vi "_VI Helpeks.vi"() -> ()   [LabVIEW 2014]
doc: "::: VI Helpeks :::\nCopyright (c) 2000-2026 Konstantin Shifershteyn. All rights reserved."
uses:
  _VIH Project Manager.llb/VIH Project Tree Typedef - Tree Item Type.ctl
  <vilib>/Utility/miscctls.llb/LVPointTypeDef.ctl
  _VIH Support Library.llb/VIH Utility - APP - Is Value Changed (BOOL).vi
  _VIH Support Library.llb/VIH Utility - APP - Is Value Changed (STR).vi
  <vilib>/Platform/browser.llb/Open URL in Default Browser (path).vi
  <vilib>/Utility/config.llb/Read Key (Path).vi
  <vilib>/Utility/config.llb/Read Key (String).vi
  <resource>/objmgr/DOMUserDefRef.rc
  <vilib>/Utility/config.llb/NI_LVConfig.lvlib
panel:
  in  "%Toolbar_VI_Doc":bool caption="VI Documentation"
  in  "%Toolbar_BuildCHMOpen":bool caption="Open Output CHM File"
  in  "%Toolbar_VI_Edit":bool caption="Edit Source File"
  in  "%Toolbar_BuildCHM":bool caption="Compiled HTML Help"
  in  "%Toolbar_BuildExplore":bool caption="Explore Build Root Folder"
  in  "%Toolbar_Paste":bool caption="Paste File Spec"
  in  "%Toolbar_Copy":bool caption="Copy File Spec"
  in  "%Toolbar_Delete":bool caption="Delete Item"
  in  "%Toolbar_AddGroup":bool caption="Add Group"
  in  "%Toolbar_AddFile":bool caption="Add File"
  in  "%Toolbar_Warning":bool caption="Warning"
  in  "%Toolbar_VI_Term":bool caption="VI Terminal Controls"
  in  "%Toolbar_VI_Open":bool caption="Open Source File"
  in  "%Toolbar_DialogRules":bool caption="Overview File Rules"
  in  "%Toolbar_DialogFiles":bool caption="Overview Project Files"
  in  "%Toolbar_BuildOpen":bool caption="Open Output Help File"
  in  "%Toolbar_BuildLog":bool caption="Open Build Log"
  in  "%Toolbar_BuildSel":bool caption="Build Selected"
  in  "%Toolbar_BuildAll":bool caption="Build All"
  in  "%Toolbar_Save":bool caption="Save Project"
  in  "%Toolbar_Open":bool caption="Open Project"
  in  "%Toolbar_New":bool caption="New Project"
  in  "%%% Show XML":bool
  in  "Tree":string[](tree) caption="Project Tree"
  out "Item Title":string caption="Item Info"
  out "Item Icon":picture
  out "Item Icon BG":string caption="Item Info"
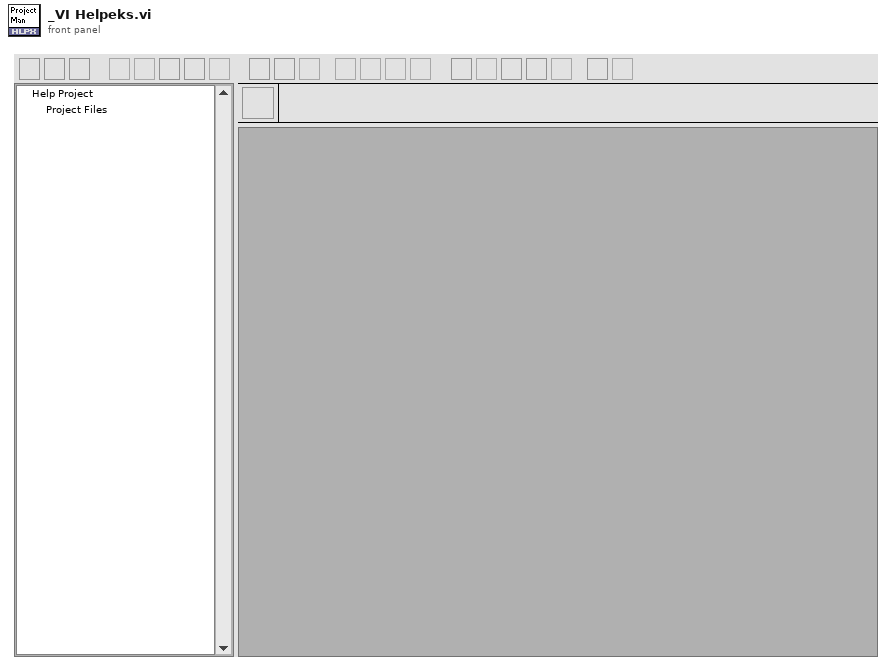
[diagram p1: front panel]
types:
  T1 = typedef "LVPointTypeDef.ctl" = cluster{"Horizontal":i16, "Vertical":i16}
  T2 = typedef "VIH Project Tree Typedef - Tree Item Type.ctl" = enum32{"<Invalid>", "Project", "Proj Files", "Proj Rules", "File Group", "Rule Group", "Any File", "LV Func", ".mnu", ".mnu (dyn)", ".vi", ".vi (dyn)", ".vit", ".vit (dyn)", ".ctl", ".ctl (dyn)", ".ctt", ".ctt (dyn)", "polyVI", "polyVI (dyn)", "expVI", "expVI (dyn)", "HTML", "PolyVI Inst"}
  T3 = cluster{"Product Name":string, "Short Name":string, "Product Version":string, "Release Timestamp":string, "Developer":string, "Copyright":string}
  T4 = enum16{"nop", "Init", "get index", "get symbols"}
  T5 = enum16{"Open", "Close", "Update", "Set Category"}
  T6 = enum32{"edit", "explore", "find", "open", "print"}
  T7 = enum32{"Bad", "Idle", "Run top level", "Running"}
  T8 = enum32{"Invalid", "Default", "Floating", "Floating/Auto-Hide", "Modal"}
  T9 = cluster{"Left Button Key Shortcut":cluster{"Control":bool, "Shift":bool, "Key":string}, "Center Button Key Shortcut":cluster{"Control":bool, "Shift":bool, "Key":string}, "Right Button Key Shortcut":cluster{"Control":bool, "Shift":bool, "Key":string}}
  T10 = enum16{"get", "get all", "set", "Init", "delete", "rename"}
  T11 = enum16{"get", "get all", "set", "Init", "delete"}
  T12 = enum8{"Enabled", "Disabled", "Disabled and Grayed Out"}
  T13 = typedef "eventvkey.ctl" = enum16{"ASCII", "Enter", "Return", "Shift", "Ctrl", "Alt", "Cmd", "Opt", "Caps", "NumLock", "Clear", "Break", "Up", "Down", "Left", "Right", "Insert", "Delete", "Home", "End", "PageUp", "PageDown", "Escape", "Help", "Pause", "ScrollLock", "F1", "F2", "F3", "F4", "F5", "F6", "F7", "F8", "F9", "F10", "F11", "F12", "F13", "F14", "F15", "F16", "F17", "F18", "F19", "F20", "F21", "F22", "F23", "F24", "Play", "VolumeUp", "VolumeDown", "Mute", "Two Byte Char"}
  T14 = cluster{"Shift":bool, "Ctrl":bool, "Alt":bool, "Cmd":bool, "Opt":bool}
  T15 = typedef "VIH HelpGen Typedef - Cluster - Group Rule.ctl" = cluster{"Source Root Dir":path, "Build Root Dir":path, "BuildHelp":T16, "Source Paths":T17, "Target Paths":T18, "VIDscrMode":T19, "MenuDscrMode":T19, "MenuItemIcons":T16, "Control Rules":T20[], "Flags":T22, "Ctl_DscrMode":T19, "Ctl_ClustMembers":T16, "Ctl_EnumValues":T16, "%Comments":string, "PVIIDscrMode":T19, "VIDetailsMode":T19, "ProductInfoMode":T16, "ProductInfoText":string}
  T16 = typedef "VIH HelpGen Typedef - Enum - Default,Enable,Disable.ctl" = enum16{"Default", "Enable", "Disable"}
  T17 = typedef "VIH HelpGen Typedef - Cluster - Group Rule - Source Paths.ctl" = cluster{"CSS Files":path[], "JS Files":path[], "VI Template":path, "Menu Template":path, "PolyVI Template":path}
  T18 = typedef "VIH HelpGen Typedef - Cluster - Group Rule - Target Paths.ctl" = cluster{"HTML Dir":path, "Image Dir":path, "CSS Dir":path, "JS Dir":path}
  T19 = typedef "VIH HelpGen Typedef - Enum - Description Mode.ctl" = enum16{"Default", "Description", "Description1", "Description2", "Custom", "None"}
  T20 = typedef "VIH HelpGen Typedef - Cluster - Control Rule.ctl" = cluster{"CtrlID":string, "CustomRule":bool, "DscrMode":T19, "Description":string, "ClusterMembers":T16, "EnumValues":T16, "EnumValDscr":T21[], "CustomName":string}
  T21 = typedef "VIH HelpGen Typedef - Cluster - Enum Value Info.ctl" = cluster{"Value":ext, "String":string, "Description":string}
  T22 = typedef "VIH HelpGen Typedef - Cluster - Group Rule - Flags.ctl" = cluster{"Override CSS Files":bool, "Override JS Files":bool, "Override Ctl Rules":bool}
  T23 = typedef "LVPoint32TypeDef.ctl" = cluster{"Horizontal":i32, "Vertical":i32}
  T24 = typedef "VIH Project Tree Typedef - Tree Refnum.ctl" = refnum<vi>
  T25 = typedef "lveventtype.ctl" = enum32{"Null", "Timeout", "Annotation Menu Selection", "Annotation Menu Selection?", "App Instance Close", "App Instance Close?", "Autoscale Range Change", "Bookmark Info Change", "Cell Edit", "Cell Edit?", "Cursor Grab", "Cursor Grab?", "Cursor Menu Selection", "Cursor Menu Selection?", "Cursor Move", "Cursor Release", "Data Change", "Direction Change", "Display State Change", "Drag Ended", "Drag Enter", "Drag Leave", "Drag Over", "Drag Source Update", "Drag Starting", "Drag Starting?", "Drop", "Exec State Change", "Key Down", "Key Down?", "Key Repeat", "Key Repeat?", "Key Up", "Listbox Double Click", "Menu Activation?", "Menu Selection (App)", "Menu Selection? (App)", "Menu Selection (User)", "Mouse Down", "Mouse Down?", "Mouse Enter", "Mouse Leave", "Mouse Move", "Mouse Up", "Mouse Wheel", "NI Security User Change (App)", "Pane Size", "Panel Close", "Panel Close?", "Panel Resize", "Plot Attribute Change", "Scale Range Change", "Shortcut Menu Activation?", "Shortcut Menu Selection (App)", "Shortcut Menu Selection? (App)", "Shortcut Menu Selection (User)", "Tree Double Click", "Tree Drag", "Tree Drag?", "Tree Drop", "Tree Drop?", "Tree Item Close", "Tree Item Close?", "Tree Item Open", "Tree Item Open?", "User Event", "Value Change"}
  T26 = cluster{"Show Window":bool, "Show Progress":bool, "Generate HTML":bool, "Generate HHP":bool, "Generate CHM":bool}
  T27 = cluster{"ShowQuickTips":bool, "NextQuickTip":i32, "FastLoadVI":bool, "EditPrgs ":cluster{"FileExtension":string, "CustProgram":path, "UseCustPrg":bool}[]}
  T28 = typedef "NI_LVConfig.lvlib/Config Data RefNum.ctl" = refnum<k1>
  T29 = cluster{"FileExtension":string, "CustProgram":path, "UseCustPrg":bool}[]
  T30 = typedef "VIH HelpGen Typedef - Cluster - File Rule.ctl" = cluster{"OutName":string, "BuildHelp":T16, "Source Paths":T31, "Target Paths":T32, "DscrMode":T19, "Description":string, "Control Rules":T20[], "Flags":T22, "Ctl_DscrMode":T19, "Ctl_ClustMembers":T16, "Ctl_EnumValues":T16, "MenuItemIcons":T16, "%Comments":string, "DetailsMode":T19, "DetailsText":string, "ProductInfoMode":T16, "ProductInfoText":string}
  T31 = typedef "VIH HelpGen Typedef - Cluster - File Rule - Source Paths.ctl" = cluster{"CSS Files":path[], "JS Files":path[], "Html Template":path}
  T32 = typedef "VIH HelpGen Typedef - Cluster - File Rule - Target Paths.ctl" = cluster{"HTML Dir":path, "Image Dir":path, "CSS Dir":path, "JS Dir":path}
  T33 = typedef "VIH HelpGen Typedef - Palette - Item Type Enum.ctl" = enum32{"<Invalid>", "<unknown>", "VI", "Menu", "LV Func", "Express VI", "Poly VI", "CTL", "HTML"}
  T34 = typedef "VIH - CHM Project - HHP Generation Params Cluster.ctl" = cluster{"HHP_Template":enum16{"default", "custom"}, "HHP_Template_CustomPath":path, "HHP_Target":enum16{"default", "custom"}, "HHP_Target_CustomPath":path, "HHP_CreateTOC":bool, "HHP_CreateIDX":bool, "HHP_DefaultTopic":enum16{"auto", "custom"}, "HHP_DefaultTopic_CustomPath":path, "CHM_Filename":path, "HHP_AutoBuild":bool, "CHM_AutoBuild":bool}
  T35 = enum16{"Left Button", "Center Button", "Right Button", "Window Close"}
  T36 = cluster{"DOM doc":refnum<k20>, "Project":refnum<k20>, "Files":refnum<k20>}
  T37 = typedef "VIH HelpGen Typedef - Product Info Cluster.ctl" = cluster{"ProductName":string, "Version":string, "Author":string, "Company":string, "Copyright":string, "Website":string, "Email":string, "AddInfo":string}
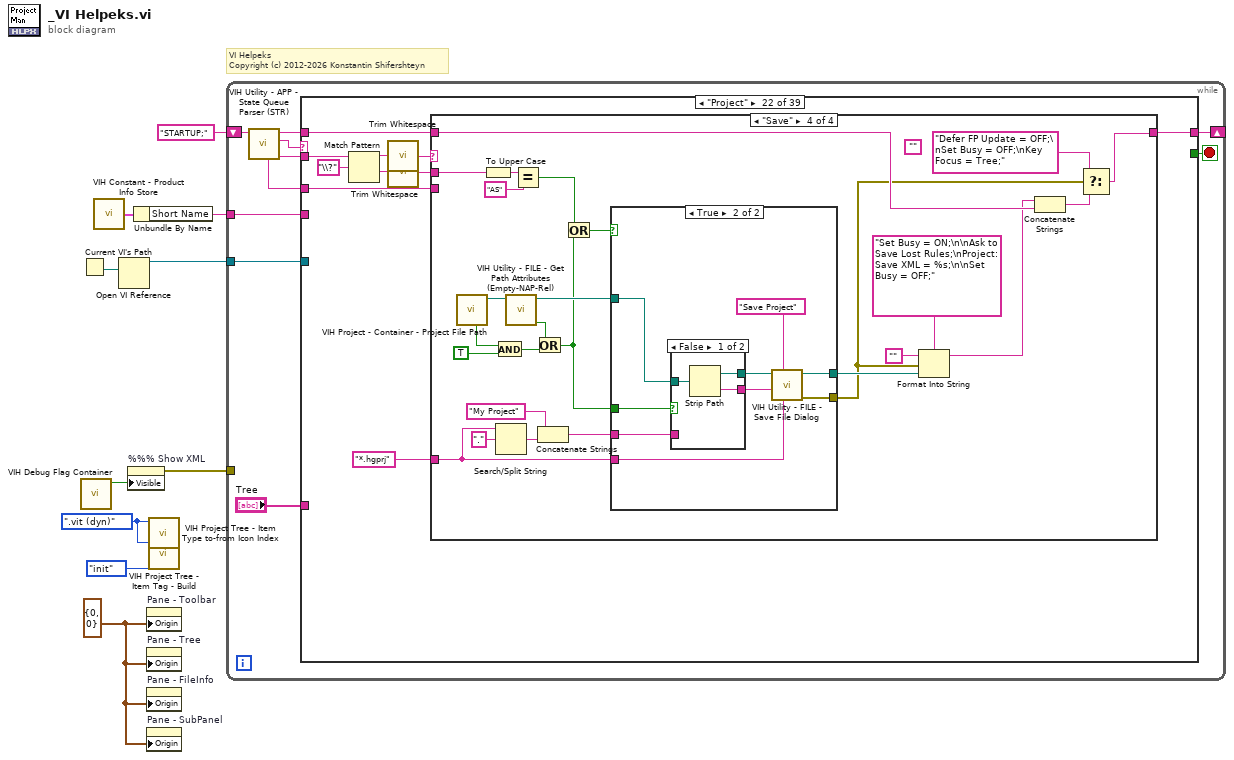
[diagram p0: block diagram]
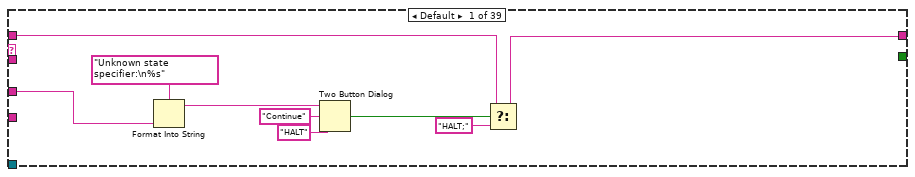
[diagram p2: hidden frame]
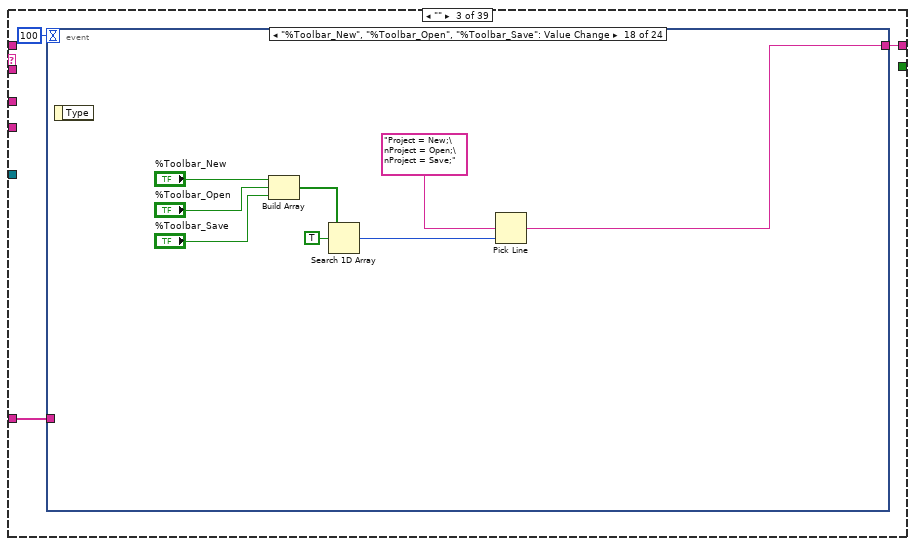
[diagram p4: hidden frame]
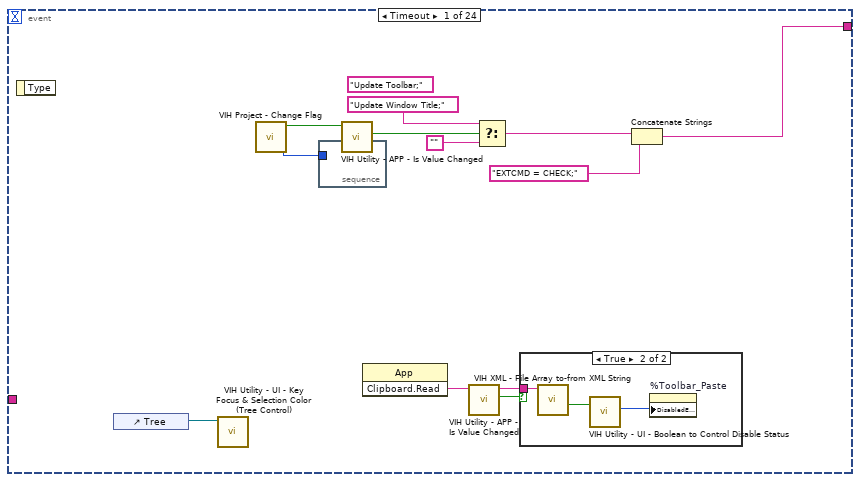
[diagram p5: hidden frame]
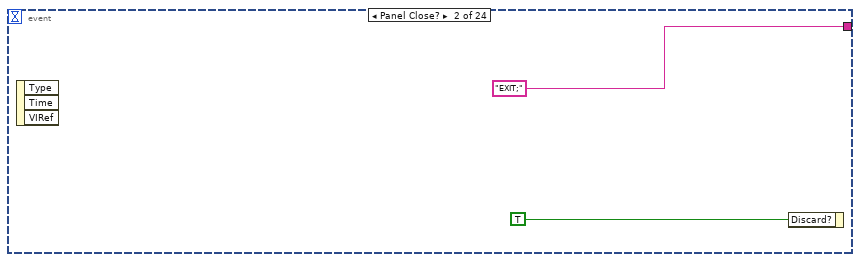
[diagram p7: hidden frame]
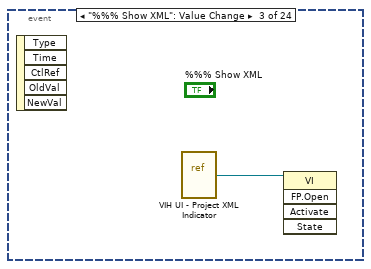
[diagram p8: hidden frame]
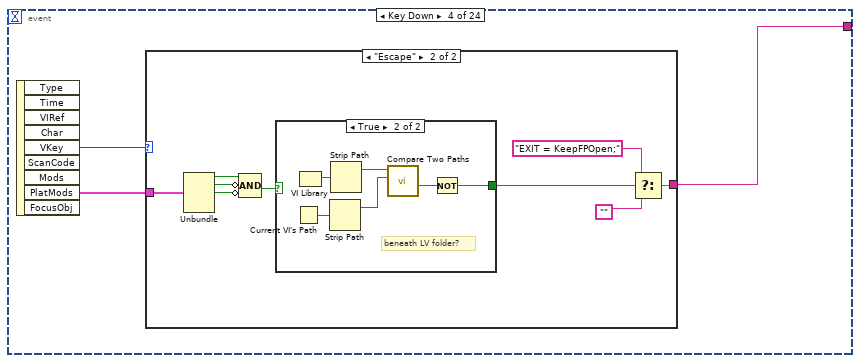
[diagram p9: hidden frame]
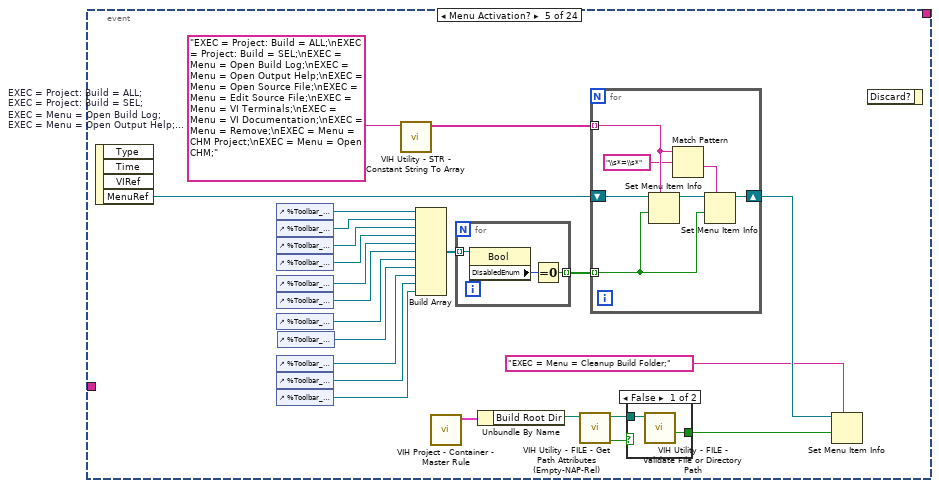
[diagram p12: hidden frame]
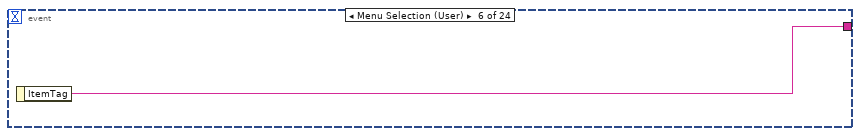
[diagram p14: hidden frame]
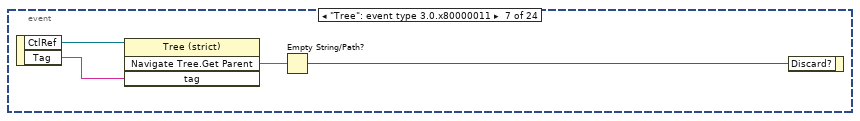
[diagram p15: hidden frame]
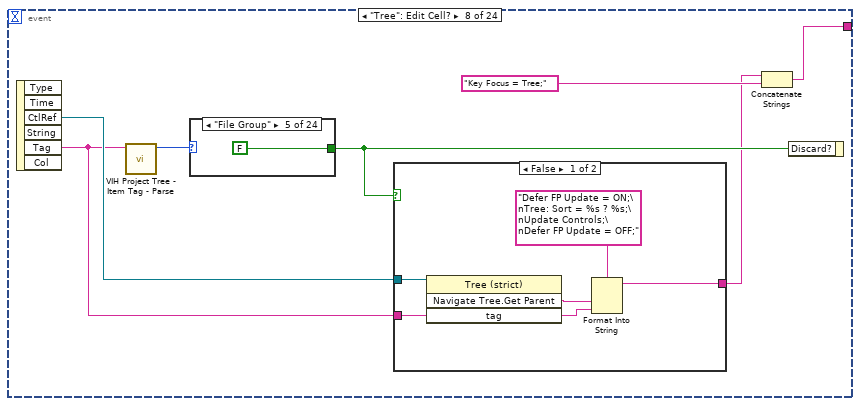
[diagram p16: hidden frame]
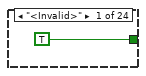
[diagram p18: hidden frame]
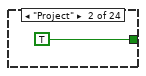
[diagram p19: hidden frame]
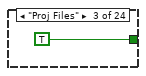
[diagram p20: hidden frame]
diagram:
  w5 = T1 {"Horizontal"=0, "Vertical"=0} ("Origin")
  w8 = VIH_Project_Tree_Typedef_-_Tree_Item_Type.".vit (dyn)" ("Item Type")
  # "VI Helpeks\nCopyright (c) 2012-2026 Konstantin Shifershteyn"
  n1 = Current VI's Path() -> (path=w2:path)
  n2 = call "VIH Debug Flag Container.vi"() -> ("Debug Mode"=w4:bool)  [unwired: 11 in]
  n3 = call "VIH Constant - Product Info Store.vi"() -> ("Product Info"=w6:T3)
  n4 = Open VI Reference(vi path=w2) -> (vi reference=w1:refnum<vi>)  [unwired: 5 in, 1 out]
  n5 = property on="%%% Show XML" class="Bool"("Visible"=w4) -> (error out=w3:errorcluster)  [unwired: 2 in, 1 out]
  n6 = Unbundle By Name(w6) -> ("Short Name"=w7:string)
  n7 = property on="Pane - Toolbar" class="Pane"("Origin"=w5) -> ()  [unwired: 2 in, 2 out]
  n8 = property on="Pane - Tree" class="Pane"("Origin"=w5) -> ()  [unwired: 2 in, 2 out]
  n9 = property on="Pane - FileInfo" class="Pane"("Origin"=w5) -> ()  [unwired: 2 in, 2 out]
  n10 = property on="Pane - SubPanel" class="Pane"("Origin"=w5) -> ()  [unwired: 2 in, 2 out]
  n11 = call "VIH Project Tree - Item Type to-from Icon Index.vi"("Item Type"=w8) -> ()  [unwired: 10 in, 1 out]
  n12 = call "VIH Project Tree - Item Tag - Build.vi"("cmd (build)"=enum16{"build", "init"}."init", "Item Type"=w8) -> ()  [unwired: 8 in, 2 out]
  n13 = while {
    shift-right: [w17] -> _
    shift-left: "STARTUP;" -> [w20]
    tunnel: w7 -> [w12]
    tunnel: w3 -> [_]
    tunnel: w1 -> [w11]
    stop <- w15 stop-if-true
    n14 = call "VIH Utility - APP - State Queue Parser (STR).vi"("input queue"=w20) -> ("state parameters"=w14:string, "state"=w19:string, "remained queue"=w16:string, "complete state specifier"=w18:string)  [unwired: 5 in]
    n15 = case shown="\"Project\"" w19 {
      tunnel: w18 -> [w28 _ _ _ _ _ _ w438 _ _ _ _ _ _ _ w624 _ _ _ _ _ w1140 _ _ _ _ _ _ _ _ _ _ _ _ _ _ _ _ _]
      tunnel: [w22 w30 w33 w364 w397 w406 w418 w437 w545 w574 w583 w598 w608 w614 w616 w623 w1082 w1086 w1091 w1109 w1135 w1137 w1209 w1215 w1285 w1329 w1340 w1351 w1473 w1491 w1502 w1551 w1570 w1580 w1595 w1605 w1615 w1666 w1719] -> w17
      tunnel: w16 -> [w23 w30 _ w365 w398 w406 w418 w436 _ w574 w583 w598 w608 w614 w616 w630 w1081 w1086 w1092 w1116 w1135 w1136 w1210 w1216 w1286 w1330 w1340 w1369 w1476 w1491 w1502 w1551 w1570 w1582 w1595 w1605 w1621 w1666 w1732]
      tunnel: [_ _ _ _ _ _ _ _ _ TRUE _ _ _ _ _ _ _ _ _ _ _ _ _ _ _ _ _ _ _ _ _ _ _ _ _ _ _ _ _] -> w15
      tunnel: w14 -> [_ _ _ _ _ w402 w416 w441 w544 w572 _ w597 w607 w612 w615 w629 w1084 _ _ _ _ w1145 w1205 w1212 w1283 w1327 w1337 w1367 _ _ _ _ w1567 _ _ _ w1616 _ w1725]
      tunnel: "Tree" -> [_ _ w31 _ _ _ _ _ _ _ _ _ _ _ _ w619 _ _ _ _ _ _ _ _ _ _ _ w1368 _ _ _ _ _ _ _ _ _ w1655 _]
      tunnel: w12 -> [_ _ _ _ _ _ _ _ _ w570 _ _ _ _ _ _ _ _ _ _ _ _ _ _ w1253 _ _ w1344 _ _ _ _ _ _ _ w1601 _ _ _]
      tunnel: w11 -> [_ _ _ _ _ w407 _ _ _ w560 _ _ _ _ _ _ _ _ _ _ _ _ _ _ _ _ _ _ _ _ _ _ _ _ _ _ _ _ _]
      frame Default {
        n16 = Format Into String(format string="Unknown state specifier:\n%s", w28) -> (resulting string=w27:string)  [unwired: 2 in, 1 out]
        n17 = Two Button Dialog(message=w27, 1:"HALT" ("F button name (\"Cancel\")"), 2:"Continue" ("T button name (\"OK\")")) -> (T button?=w24:bool)
        n18 = Select(t=w23, s=w24, f="HALT;") -> (s? t:f=w22:string)
      }
      frame "#" {
      }
      frame "" {
        n19 = event shown="[17] \"%Toolbar_New\", \"%Toolbar_Open\", \"%Toolbar_Save\": Value Change" {
          selector: _ -> [_ _ _ _ _ _ _ _ _ _ _ _ _ _ _ _ _ _ _ _ _ _ _ _]
          dyn-events: _ -> [_ _ _ _ _ _ _ _ _ _ _ _ _ _ _ _ _ _ _ _ _ _ _ _]
          timeout: 100 -> [_ _ _ _ _ _ _ _ _ _ _ _ _ _ _ _ _ _ _ _ _ _ _ _]
          tunnel: [w35 "EXIT;" _ w52 _ w105 _ w110 _ _ w195 "Defer FP Update = ON;\nUpdate Controls;\nDefer FP Update = OFF;" ("format string") "Update Controls;\nKey Focus = Tree;" w260 "Key Focus = Tree;" ("format string") w279 w281 w307 w316 w327 w336 w343 w353 "Menu = WARNING;"] -> w33
          tunnel: w31 -> [_ _ _ _ _ _ _ _ _ _ _ _ _ _ _ _ _ _ _ _ _ _ _ _]
          event Timeout {
            (unwired) "Update Toolbar;"
            n20 = event-data() -> ()  [unwired: 1 in, 1 out]
            n21 = control-ref of="Tree"() -> (w45:refnum<vi>)
            n22 = call "VIH Utility - UI - Key Focus & Selection Color (Tree Control).vi"("Tree Refnum"=w45) -> ()  [unwired: 8 in, 3 out]
            n23 = call "VIH Project - Change Flag.vi"() -> ("Counter"=w39:i32, "Flag"=w40:bool)  [unwired: 10 in]
            n24 = stacked-sequence {
              tunnel: w39 -> [_]
              frame #0 {
              }
            }
            n25 = call-poly "VIH Utility - APP - Is Value Changed.vi"("Value"=w40) -> ("Changed"=w44:bool)  [unwired: 5 in, 1 out]
            n26 = invoke class="App" method="Clipboard.Read"() -> ("Read Clipbrd"=w36:string)  [unwired: 3 in, 2 out]
            n27 = call-poly "VIH Utility - APP - Is Value Changed.vi"("Value"=w36) -> ("Changed"=w38:bool, "dup Value"=w37:string)  [unwired: 5 in]
            n28 = Select(t="Update Window Title;", s=w44, f="") -> (s? t:f=w41:string)
            n29 = case shown="True" w38 {
              tunnel: w37 -> [_ w46]
              frame False {
              }
              frame True {
                n30 = call "VIH XML - File Array to-from XML String.vi"("XML in"=w46) -> ("available"=w47:bool)  [unwired: 7 in, 3 out]
                n31 = call "VIH Utility - UI - Boolean to Control Disable Status.vi"("Status in"=w47) -> ("Control Disable if False"=w48:u8)  [unwired: 3 in, 1 out]
                n32 = property on="%Toolbar_Paste" class="Bool"("DisabledEnum"=w48) -> ()  [unwired: 2 in, 2 out]
              }
            }
            n33 = Concatenate Strings(w41, "EXTCMD = CHECK;") -> (w35:string)
          }
          event Panel Close? {
            n34 = event-data() -> ()  [unwired: 1 in, 3 out]
            n35 = event-data("Discard?"=TRUE) -> ()  [unwired: 1 in, 1 out]
          }
          event "%%% Show XML": Value Change {
            n36 = event-data() -> ()  [unwired: 1 in, 5 out]
            n37 = vi-ref "VIH UI - Project XML Indicator.vi"() -> (w51:refnum<vi>)
            n38 = invoke class="VI" method="FP.Open"(reference=w51) -> ()  [unwired: 4 in, 5 out]
          }
          event Key Down {
            n39 = event-data() -> ("VKey"=w54:T13, "PlatMods"=w53:T14)  [unwired: 1 in, 7 out]
            n40 = case shown="\"Escape\"" w54 {
              tunnel: w53 -> [_ w63]
              tunnel: [_ w57] -> w52
              frame Default {
              }
              frame "Escape" {
                n41 = Unbundle(w63) -> ("Shift"=w62:bool, "Ctrl"=w61:bool, "Alt"=w60:bool)  [unwired: 2 out]
                n42 = Compound Arithmetic op=AND(w62, invert w61, invert w60) -> (w55:bool)
                n43 = case shown="True" w55 {
                  tunnel: [_ w64] -> w56
                  frame False {
                  }
                  frame True {
                    # "beneath LV folder?"
                    n44 = Current VI's Path() -> (path=w66:path)
                    n45 = VI Library() -> (path=w69:path)
                    n46 = Strip Path(path=w66) -> (stripped path=w67:path)  [unwired: 1 out]
                    n47 = Strip Path(path=w69) -> (stripped path=w68:path)  [unwired: 1 out]
                    n48 = call <vilib>:"Compare Two Paths.vi"("Path 2"=w67, "Path 1"=w68) -> ("Path 2 Relative to Path 1?"=w65:bool)  [unwired: 6 in, 3 out]
                    n49 = Not(x=w65) -> (.not. x?=w64:bool)
                  }
                }
                n50 = Select(t="EXIT = KeepFPOpen;", s=w56, f="") -> (s? t:f=w57:string)
              }
            }
          }
          event Menu Activation? {
            w85 = "EXEC = Project: Build = ALL;\nEXEC = Project: Build = SEL;\nEXEC = Menu = Open Build Log;\nEXEC = Menu = Open Output Help;\nEXEC = Menu = Open Source File;\nEXEC = Menu = Edit Source File;\nEXEC = Menu = VI Terminals;\nEXEC = Menu = VI Documentation;\nEXEC = Menu = Remove;\nEXEC = Menu = CHM Project;\nEXEC = Menu = Open CHM;"  # EXEC = Project: Build = ALL; EXEC = Project: Build = SEL; EXEC = Menu = Open Build Log; EXEC = Menu = Open Output Help; EXEC = Menu = Open Source File; EXEC = Menu = Edit Source File; EXEC = Menu = VI Terminals; EXEC = Menu = VI Documentation; EXEC = Menu = Remove; EXEC = Menu = CHM Project; EXEC = Menu = Open CHM;
            n51 = event-data() -> ("MenuRef"=w92:refnum<k9>)  [unwired: 1 in, 3 out]
            n52 = control-ref of="%Toolbar_BuildAll"() -> (w91:refnum<vi>)
            n53 = control-ref of="%Toolbar_BuildSel"() -> (w90:refnum<vi>)
            n54 = control-ref of="%Toolbar_BuildLog"() -> (w89:refnum<vi>)
            n55 = control-ref of="%Toolbar_BuildOpen"() -> (w88:refnum<vi>)
            n56 = control-ref of="%Toolbar_VI_Open"() -> (w87:refnum<vi>)
            n57 = control-ref of="%Toolbar_VI_Edit"() -> (w72:refnum<vi>)
            n58 = control-ref of="%Toolbar_VI_Term"() -> (w86:refnum<vi>)
            n59 = control-ref of="%Toolbar_Delete"() -> (w82:refnum<vi>)
            n60 = control-ref of="%Toolbar_BuildCHM"() -> (w80:refnum<vi>)
            n61 = control-ref of="%Toolbar_BuildCHMOpen"() -> (w71:refnum<vi>)
            n62 = control-ref of="%Toolbar_VI_Doc"() -> (w70:refnum<vi>)
            n63 = call "VIH Utility - STR - Constant String To Array.vi"("String in"=w85) -> ("Array out"=w84:string[])  [unwired: 10 in]
            n64 = Build Array(w91, w90, w89, w88, w87, w72, w86, w70, w82, w80, w71) -> (w83:refnum<vi>[])
            n65 = call "VIH Project - Container - Master Rule.vi"() -> ("Rule out"=w76:T15)  [unwired: 11 in]
            n66 = for {
              tunnel: w83 -> [w96] mode=indexing
              tunnel: [w95] -> w81 mode=indexing
              n67 = property class="Bool"(reference=w96) -> ("DisabledEnum"=w97:T12)  [unwired: 1 in, 2 out]
              n68 = Equal To 0?(x=w97) -> (x = 0?=w95:bool)
            }
            n69 = Unbundle By Name(w76) -> ("Build Root Dir"=w77:path)
            n70 = call "VIH Utility - FILE - Get Path Attributes (Empty-NAP-Rel).vi"("Path"=w77) -> ("Not A Path or Empty path"=w79:bool, "dup Path"=w78:path)  [unwired: 6 in, 3 out]
            n71 = for {
              tunnel: w84 -> [w102] mode=indexing
              tunnel: w81 -> [w99] mode=indexing
              shift-right: [w98] -> w75
              shift-left: w92 -> [w104]
              n72 = Set Menu Item Info(7:w102, 9:w99, 11:w104) -> (3:w103:refnum<k9>)  [unwired: 4 in, 1 out]
              n73 = Match Pattern(string=w102, regular expression="\\s*=\\s*") -> (after substring=w100:string)  [unwired: 1 in, 3 out]
              n74 = Set Menu Item Info(7:w100, 9:w99, 11:w103) -> (3:w98:refnum<k9>)  [unwired: 4 in, 1 out]
            }
            n75 = case shown="False" w79 {
              tunnel: w78 -> [w94 _]
              tunnel: [w93 _] -> w73
              frame False {
                n76 = call "VIH Utility - FILE - Validate File or Directory Path.vi"("Path"=w94) -> ("directory"=w93:bool)  [unwired: 6 in, 4 out]
              }
              frame True {
              }
            }
            n77 = Set Menu Item Info(7:"EXEC = Menu = Cleanup Build Folder;", 9:w73, 11:w75) -> ()  [unwired: 4 in, 2 out]
            n78 = event-data() -> ()  [unwired: 2 in, 1 out]
          }
          event Menu Selection (User) {
            n79 = event-data() -> ("ItemTag"=w105:string)  [unwired: 1 in]
          }
          event "Tree": event type 3.0.x80000011 {
            n80 = event-data() -> ("CtlRef"=w109:refnum<vi>, "Tag"=w108:string)  [unwired: 1 in]
            n81 = invoke class="Tree (strict)" method="Navigate Tree.Get Parent"(reference=w109, "tag"=w108) -> ("Navigate Tree:Get Parent"=w107:string)  [unwired: 2 in, 3 out]
            n82 = Empty String/Path?(string/path=w107) -> (empty?=w106:bool)
            n83 = event-data("Discard?"=w106) -> ()  [unwired: 1 in, 1 out]
          }
          event "Tree": Edit Cell? {
            n84 = event-data() -> ("CtlRef"=w114:refnum<vi>, "Tag"=w113:string)  [unwired: 1 in, 4 out]
            n85 = call "VIH Project Tree - Item Tag - Parse.vi"("Tree Item Tag"=w113) -> ("Item Type"=w116:T2)  [unwired: 8 in, 2 out]
            n86 = case shown="\"File Group\"" w116 {
              tunnel: [TRUE TRUE TRUE TRUE FALSE FALSE TRUE TRUE TRUE TRUE TRUE TRUE TRUE TRUE TRUE TRUE TRUE TRUE TRUE TRUE TRUE TRUE TRUE TRUE] -> w115
              frame "<Invalid>" {
              }
              frame "Project" {
              }
              frame "Proj Files" {
              }
              frame "Proj Rules" {
              }
              frame "File Group" {
              }
              frame "Rule Group" {
              }
              frame "Any File" {
              }
              frame "LV Func" {
              }
              frame ".mnu" {
              }
              frame ".mnu (dyn)" {
              }
              frame ".vi" {
              }
              frame ".vi (dyn)" {
              }
              frame ".vit" {
              }
              frame ".vit (dyn)" {
              }
              frame ".ctl" {
              }
              frame ".ctl (dyn)" {
              }
              frame ".ctt" {
              }
              frame ".ctt (dyn)" {
              }
              frame "polyVI" {
              }
              frame "polyVI (dyn)" {
              }
              frame "expVI" {
              }
              frame "expVI (dyn)" {
              }
              frame "HTML" {
              }
              frame "PolyVI Inst" {
              }
            }
            n87 = case shown="False" w115 {
              tunnel: w114 -> [w121 _]
              tunnel: w113 -> [w117 _]
              tunnel: [w118 _] -> w111
              frame False {
                n88 = invoke class="Tree (strict)" method="Navigate Tree.Get Parent"(reference=w121, "tag"=w117) -> ("Navigate Tree:Get Parent"=w119:string)  [unwired: 2 in, 3 out]
                n89 = Format Into String(format string="Defer FP Update = ON;\nTree: Sort = %s ? %s;\nUpdate Controls;\nDefer FP Update = OFF;", w119, w117) -> (resulting string=w118:string)  [unwired: 2 in, 1 out]
              }
              frame True {
              }
            }
            n90 = Concatenate Strings(w111, "Key Focus = Tree;") -> (w110:string)
            n91 = event-data("Discard?"=w115) -> ()  [unwired: 1 in, 1 out]
          }
          event "Tree": Drag Starting? {
            n92 = event-data() -> ("CtlRef"=w149:refnum<vi>)  [unwired: 1 in, 8 out]
            n93 = property class="Tree (strict)"(reference=w149) -> ("Value"=w146:string[])  [unwired: 1 in, 2 out]
            n94 = for {
              tunnel: [w154] -> w150 mode=indexing
              tunnel: w146 -> [w153] mode=indexing
              n95 = call "VIH Project Tree - Item Tag - Parse.vi"("Tree Item Tag"=w153) -> ("Item File Path"=w151:path, "Item Type"=w152:T2)  [unwired: 8 in, 1 out]
              n96 = case shown="\"PolyVI Inst\"" w152 {
                tunnel: [w155 FALSE FALSE FALSE TRUE TRUE TRUE FALSE TRUE FALSE TRUE FALSE TRUE FALSE TRUE FALSE TRUE FALSE TRUE FALSE TRUE FALSE TRUE FALSE] -> w154
                tunnel: w151 -> [w157 _ _ _ _ _ _ _ _ _ _ _ _ _ _ _ _ _ _ _ _ _ _ _]
                frame "<Invalid>" {
                  (unwired) FALSE
                  n97 = Empty String/Path?(string/path=w157) -> (empty?=w156:bool)
                  n98 = Not(x=w156) -> (.not. x?=w155:bool)
                }
                frame "Project" {
                }
                frame "Proj Files" {
                }
                frame "Proj Rules" {
                }
                frame "File Group" {
                }
                frame "Rule Group" {
                }
                frame "Any File" {
                }
                frame "LV Func" {
                }
                frame ".mnu" {
                }
                frame ".mnu (dyn)" {
                }
                frame ".vi" {
                }
                frame ".vi (dyn)" {
                }
                frame ".vit" {
                }
                frame ".vit (dyn)" {
                }
                frame ".ctl" {
                }
                frame ".ctl (dyn)" {
                }
                frame ".ctt" {
                }
                frame ".ctt (dyn)" {
                }
                frame "polyVI" {
                }
                frame "polyVI (dyn)" {
                }
                frame "expVI" {
                }
                frame "expVI (dyn)" {
                }
                frame "HTML" {
                }
                frame "PolyVI Inst" {
                }
              }
            }
            n99 = And Array Elements(Boolean array=w150) -> (logical AND=w148:bool)
            n100 = Not(x=w148) -> (.not. x?=w147:bool)
            n101 = event-data("Discard?"=w147) -> ()  [unwired: 1 in, 1 out]
          }
          event "Tree": event type 3.0.xa000003a {
            n102 = event-data() -> ("CtlRef"=w188:refnum<vi>, "Coords"=w189:T23)  [unwired: 1 in, 3 out]
            n103 = invoke class="Tree (strict)" method="Point To Row Column"(reference=w188, "Point"=w189) -> (reference out=w187:refnum<vi>, "InBounds"=w182:bool, "Tag"=w184:string)  [unwired: 6 in, 5 out]
            n104 = property class="Tree (strict)"(reference=w187) -> (reference out=w186:refnum<vi>, "Value"=w185:string[])  [unwired: 1 in, 1 out]
            n105 = call "VIH Project Tree - Is Drop Allowed.vi"("Target Item Tag"=w184, "Source Item Tags"=w185, "Tree Refnum"=w186) -> ("Drop Allowed"=w183:bool)  [unwired: 6 in, 2 out]
            n106 = And(x=w183, y=w182) -> (x .and. y?=w181:bool)
            n107 = event-data("Accepted?"=w181) -> ()  [unwired: 1 in, 1 out]
          }
          event "Tree": Drop {
            n108 = event-data() -> ("CtlRef"=w197:refnum<vi>, "Coords"=w198:T23)  [unwired: 1 in, 3 out]
            n109 = invoke class="Tree (strict)" method="Point To Row Column"(reference=w197, "Point"=w198) -> (reference out=w193:refnum<vi>, "Tag"=w192:string)  [unwired: 6 in, 6 out]
            n110 = property class="Tree (strict)"(reference=w193) -> (reference out=w194:refnum<vi>, "Value"=w190:string[])  [unwired: 1 in, 1 out]
            n111 = call "VIH Project Tree - Is Drop Allowed.vi"("Target Item Tag"=w192, "Source Item Tags"=w190, "Tree Refnum"=w194) -> ("Drop Allowed"=w191:bool)  [unwired: 6 in, 2 out]
            n112 = case shown="True" w191 {
              tunnel: w197 -> [_ w201]
              tunnel: w192 -> [_ w204]
              tunnel: [_ w205] -> w195
              tunnel: w190 -> [_ w203]
              frame False {
              }
              frame True {
                n113 = call "VIH Project Tree - Defer Panel Updates.vi"("Defer Panel Updates (F)"=TRUE, "Project Tree"=w201) -> ("dup Project Tree"=w200:T24)  [unwired: 7 in, 2 out]
                n114 = Index Array(array=w203) -> (element=w202:string)  [unwired: 1 in]
                n115 = for {
                  tunnel: w204 -> [w210]
                  shift-right: [w211] -> w207
                  shift-left: w200 -> [w213]
                  tunnel: w203 -> [w209] mode=indexing
                  n116 = invoke class="Tree (strict)" method="Edit Tree Items.Move Item"(reference=w213, "tag"=w209, "New Parent"=w210, "Carry Children"=TRUE) -> (reference out=w211:T24)  [unwired: 3 in, 6 out]
                }
                n117 = invoke class="Tree (strict)" method="Open/Close.Item"(reference=w207, "tag"=w204, "Open"=TRUE) -> ()  [unwired: 2 in, 5 out]
                n118 = Format Into String(format string="Defer FP Update = ON;\nTree: Sort = %s ? %s;\nUpdate Controls;\nDefer FP Update = OFF;", w204, w202) -> (resulting string=w205:string)  [unwired: 2 in, 1 out]
              }
            }
            n119 = event-data("Accepted?"=FALSE) -> ()  [unwired: 1 in, 1 out]
          }
          event "Tree": Value Change {
            n120 = event-data() -> ("CtlRef"=w217:refnum<vi>, "NewVal"=w216:string[])  [unwired: 1 in, 3 out]
            n121 = Array Size(array=w216) -> (size(s)=w214:i32)
            n122 = case shown="2.." w214 {
              selector: w214 -> [_ w218]
              tunnel: w217 -> [_ w224]
              tunnel: w216 -> [_ w223]
              frame ..1 {
              }
              frame 2.. {
                n123 = Decrement(x=w218) -> (x-1=w222:i32)
                n124 = Index Array(array=w223, index=w222) -> (element=w219:string)
                n125 = property class="Tree (strict)"(reference=w224, "Active Item Tag"=w219) -> (reference out=w220:refnum<vi>, "Indent Level"=w221:i32)  [unwired: 1 in, 1 out]
                n126 = case shown="0, 1" w221 {
                  tunnel: w220 -> [w227 _]
                  tunnel: w219 -> [w226 _]
                  frame 0, 1 {
                    n127 = Build Array(w226) -> (w225:string[])
                    n128 = property class="Tree (strict)"(reference=w227, "Value"=w225) -> ()  [unwired: 1 in, 2 out]
                  }
                  frame Default {
                  }
                }
              }
            }
          }
          event "Tree": Shortcut Menu Activation? {
            (unwired) "Key Focus = Tree;"
            n129 = event-data() -> ("Type"=w230:T25, "CtlRef"=w238:refnum<vi>, "MenuRef"=w237:refnum<k9>, "Coords"=w229:T23)  [unwired: 1 in, 1 out]
            n130 = invoke class="Tree (strict)" method="Point To Row Column"(reference=w238, "Point"=w229) -> (reference out=w231:refnum<vi>, "InBounds"=w235:bool, "Tag"=w234:string)  [unwired: 6 in, 5 out]
            n131 = Select(t=w234, s=w235, f="") -> (s? t:f=w232:string)
            n132 = case shown="Default" w232 {
              selector: w232 -> [w243 _]
              tunnel: w237 -> [w244 _]
              tunnel: [_ TRUE] -> w236
              tunnel: w231 -> [w240 _]
              tunnel: w230 -> [w245 _]
              tunnel: w229 -> [w242 _]
              frame Default {
                n133 = property class="Tree (strict)"(reference=w240) -> (reference out=w246:refnum<vi>, "Value"=w248:string[])  [unwired: 1 in, 1 out]
                n134 = Search 1D Array(1D array=w248, element=w243) -> (index of element=w247:i32)  [unwired: 1 in]
                n135 = case shown="..-1" w247 {
                  tunnel: w246 -> [w252 w253]
                  tunnel: w243 -> [w251 _]
                  tunnel: [w249 w253] -> w239
                  frame ..-1 {
                    n136 = Build Array(w251) -> (w250:string[])
                    n137 = property class="Tree (strict)"(reference=w252, "Value"=w250) -> (reference out=w249:refnum<vi>)  [unwired: 1 in, 1 out]
                  }
                  frame 0.. {
                  }
                }
                n138 = call "VIH Project Tree - Shortcut Menu Handler.vi"("Menu Tag"="", "Coords"=w242, "MenuRef"=w244, "Project Tree"=w239, "Event Type"=w245) -> ()  [unwired: 6 in, 1 out]
              }
              frame "", "TREE_COLUMN_HEADERS" {
              }
            }
            n139 = event-data("Discard?"=w236) -> ()  [unwired: 1 in, 1 out]
          }
          event "Tree": Shortcut Menu Selection (User) {
            (unwired) "Defer FP Update = ON;\n%s\nUpdate Controls;\nDefer FP Update = OFF;\n\nKey Focus = Tree;" ("format string")
            # "Update Controls is done twice!"
            n140 = event-data() -> ("Type"=w265:T25, "CtlRef"=w266:refnum<vi>, "ItemTag"=w264:string, "Coords"=w263:T23)  [unwired: 1 in, 3 out]
            n141 = flat-sequence {
              tunnel: w263 -> [w267]
              tunnel: w264 -> [w268]
              tunnel: w265 -> [w269]
              tunnel: w266 -> [w270]
              tunnel: [w270] -> w259
              tunnel: [w269] -> w258
              tunnel: [w268] -> w257
              tunnel: [w267] -> w256
              tunnel: w259 -> [w276]
              tunnel: w258 -> [w275]
              tunnel: w257 -> [w274]
              tunnel: w256 -> [w273]
              tunnel: [w271] -> w255
              tunnel: [w277] -> w261
              tunnel: w255 -> [w277]
              frame #0 {
                n142 = call <vilib>:"Set Busy.vi"() -> ()  [unwired: 10 in, 2 out]
              }
              frame #1 {
                n143 = call "VIH Project Tree - Shortcut Menu Handler.vi"("Menu Tag"=w274, "Coords"=w273, "MenuRef"=refnum<k9> refnum, "Project Tree"=w276, "Event Type"=w275) -> ("States spec"=w271:string)  [unwired: 6 in]
              }
              frame #2 {
                n144 = call <vilib>:"Unset Busy.vi"() -> ()  [unwired: 11 in, 1 out]
              }
            }
            n145 = Format Into String(format string="Set Busy = ON;\nKey Focus = Tree;\n\nDefer FP Update = ON;\n%s\n#= Update Controls;\nDefer FP Update = OFF;\n\nSet Busy = OFF;\nKey Focus = Tree;", w261) -> (resulting string=w260:string)  [unwired: 2 in, 1 out]
          }
          event "Tree": event #0x44 {
            n146 = event-data() -> ()  [unwired: 1 in, 1 out]
          }
          event "Tree": Mouse Up {
            n147 = event-data() -> ()  [unwired: 1 in, 1 out]
            n148 = disable-structure shown="Disabled" {
              disable-tunnel: ["Key Focus = Tree;" ("format string") _] -> w279
              frame Disabled {
              }
              frame Enabled {
              }
            }
          }
          event "Tree": Key Down? {
            n149 = event-data() -> ("VKey"=w284:T13, "PlatMods"=w283:T14)  [unwired: 1 in, 7 out]
            n150 = case shown="\"Insert\"" w284 {
              tunnel: w283 -> [_ w294 w305]
              tunnel: [_ w285 w301] -> w282
              tunnel: [_ w288 w303] -> w281
              frame Default {
              }
              frame "Delete" {
                n151 = property on="%Toolbar_Delete" class="Bool"() -> ("DisabledEnum"=w287:T12)  [unwired: 2 in, 2 out]
                n152 = Unbundle(w294) -> ("Shift"=w293:bool, "Ctrl"=w292:bool, "Alt"=w291:bool)  [unwired: 2 out]
                n153 = Equal To 0?(x=w287) -> (x = 0?=w286:bool)
                n154 = Compound Arithmetic op=OR(invert w293, invert w292, invert w291) -> (w285:bool)
                n155 = And(x=w285, y=w286) -> ()  [unwired: 1 out]
                n156 = Select(t="EXEC = Menu = Remove;", s=w285, f="") -> (s? t:f=w288:string)
              }
              frame "Insert" {
                n157 = Unbundle(w305) -> ("Shift"=w298:bool, "Ctrl"=w297:bool, "Alt"=w302:bool)  [unwired: 2 out]
                n158 = Or(x=w298, y=w297) -> (x .or. y?=w296:bool)
                n159 = Not(x=w302) -> (.not. x?=w301:bool)
                n160 = Select(t="EXEC = Menu = Add Group;", s=w296, f="EXEC = Menu = Add File ? MISC;") -> (s? t:f=w300:string)
                n161 = Select(t=w300, s=w301, f="") -> (s? t:f=w303:string)
              }
            }
            n162 = event-data("Discard?"=w282) -> ()  [unwired: 1 in, 1 out]
          }
          event "%Toolbar_New", "%Toolbar_Open", "%Toolbar_Save": Value Change {
            n163 = event-data() -> ()  [unwired: 1 in, 1 out]
            n164 = Build Array("%Toolbar_New", "%Toolbar_Open", "%Toolbar_Save") -> (w310:bool[])
            n165 = Search 1D Array(1D array=w310, element=TRUE) -> (index of element=w309:i32)  [unwired: 1 in]
            n166 = Pick Line(multi-line string="Project = New;\nProject = Open;\nProject = Save;", line index=w309) -> (output string=w307:string)  [unwired: 1 in]
          }
          event "%Toolbar_BuildAll", "%Toolbar_BuildSel", "%Toolbar_BuildLog", "%Toolbar_BuildOpen", "%Toolbar_BuildExplore": Value Change {
            w321 = "EXEC = Project: Build = ALL;\nEXEC = Project: Build = SEL;\nEXEC = Menu = Open Build Log;\nEXEC = Menu = Open Output Help;\nEXEC = Menu = Explore Build Root;"  # EXEC = Project: Build = ALL; EXEC = Project: Build = SEL; EXEC = Menu = Open Build Log; EXEC = Menu = Open Output Help; EXEC = Menu = Explore Build Root;
            n167 = event-data() -> ()  [unwired: 1 in, 1 out]
            n168 = Build Array("%Toolbar_BuildAll", "%Toolbar_BuildSel", "%Toolbar_BuildLog", "%Toolbar_BuildOpen", "%Toolbar_BuildExplore") -> (w323:bool[])
            n169 = Search 1D Array(1D array=w323, element=TRUE) -> (index of element=w322:i32)  [unwired: 1 in]
            n170 = Pick Line(multi-line string=w321, line index=w322) -> (output string=w316:string)  [unwired: 1 in]
          }
          event "%Toolbar_VI_Open", "%Toolbar_VI_Term", "%Toolbar_VI_Edit", "%Toolbar_VI_Doc": Value Change {
            n171 = event-data() -> ()  [unwired: 1 in, 1 out]
            n172 = Build Array("%Toolbar_VI_Open", "%Toolbar_VI_Edit", "%Toolbar_VI_Term", "%Toolbar_VI_Doc") -> (w332:bool[])
            n173 = Search 1D Array(1D array=w332, element=TRUE) -> (index of element=w331:i32)  [unwired: 1 in]
            n174 = Pick Line(multi-line string="EXEC = Menu = Open Source File;\nEXEC = Menu = Edit Source File;\nEXEC = Menu = VI Terminals;\nEXEC = Menu = VI Documentation;", line index=w331) -> (output string=w327:string)  [unwired: 1 in]
          }
          event "%Toolbar_BuildCHM", "%Toolbar_BuildCHMOpen": Value Change {
            n175 = event-data() -> ()  [unwired: 1 in, 1 out]
            n176 = Build Array("%Toolbar_BuildCHM", "%Toolbar_BuildCHMOpen") -> (w339:bool[])
            n177 = Search 1D Array(1D array=w339, element=TRUE) -> (index of element=w338:i32)  [unwired: 1 in]
            n178 = Pick Line(multi-line string="EXEC = Menu = CHM Project;\nEXEC = Menu = Open CHM;", line index=w338) -> (output string=w336:string)  [unwired: 1 in]
          }
          event "%Toolbar_AddFile", "%Toolbar_AddGroup", "%Toolbar_Delete", "%Toolbar_Copy", "%Toolbar_Paste": Value Change {
            n179 = event-data() -> ()  [unwired: 1 in, 1 out]
            n180 = Build Array("%Toolbar_AddFile", "%Toolbar_AddGroup", "%Toolbar_Delete", "%Toolbar_Copy", "%Toolbar_Paste") -> (w351:bool[])
            n181 = Search 1D Array(1D array=w351, element=TRUE) -> (index of element=w350:i32)  [unwired: 1 in]
            n182 = Pick Line(multi-line string="EXEC = Menu = Add File ? MISC;\nEXEC = Menu = Add Group;\nEXEC = Menu = Remove;\nEXEC = Menu = Copy File Spec;\nEXEC = Menu = Paste File Spec;", line index=w350) -> (output string=w345:string)  [unwired: 1 in]
            n183 = Format Into String(format string="Defer FP Update = ON;\n%s\nDefer FP Update = OFF;", w345) -> (resulting string=w343:string)  [unwired: 2 in, 1 out]
          }
          event "%Toolbar_DialogFiles", "%Toolbar_DialogRules": Value Change {
            n184 = event-data() -> ()  [unwired: 1 in, 1 out]
            n185 = Build Array("%Toolbar_DialogFiles", "%Toolbar_DialogRules") -> (w358:bool[])
            n186 = Search 1D Array(1D array=w358, element=TRUE) -> (index of element=w357:i32)  [unwired: 1 in]
            n187 = Pick Line(multi-line string="EXEC = Menu = File List;\nEXEC = Menu = Rule List;", line index=w357) -> (output string=w353:string)  [unwired: 1 in]
          }
          event "%Toolbar_Warning": Value Change {
            n188 = event-data() -> ()  [unwired: 1 in, 1 out]
          }
        }
      }
      frame "STARTUP" {
        n189 = control-ref of="Tree"() -> (w361:refnum<vi>)
        n190 = call "VIH ExtCmd - Params Store.vi"("cmd (get)"=enum16{"Init", "get", "set", "getcfg"}."Init") -> ()  [unwired: 9 in, 2 out]
        n191 = disable-structure shown="Disabled" {
          disable-tunnel: "Utility - Set Project Tree & List Icons.vi" ("Utility VI Name") -> [w374 _]
          disable-tunnel: w361 -> [w373 _]
          frame Disabled {
            n192 = call "VIH Utility - DEV - Get DevTime Utility VIs Folder.vi"("Utility VI Name"=w374) -> ("error out"=w379:errorcluster, "Utility VIs Path"=w378:path)  [unwired: 8 in, 1 out]
            n193 = Open VI Reference(type specifier VI Refnum (for type only)=refnum<vi> refnum, vi path=w378, error in (no error)=w379) -> (vi reference=w381:refnum<vi>, error out=w382:errorcluster)  [unwired: 3 in]
            n194 = call-by-ref "?"(reference=w381, error in=w382, "Project Tree"=w373) -> (reference out=w376:refnum<vi>, error out=w377:errorcluster, "error out (Tree)"=w372:errorcluster)  [unwired: 9 in, 1 out]
            n195 = Close Reference(reference=w376, error in (no error)=w377) -> (error out=w371:errorcluster)
            n196 = Select(t=w371, s=w371, f=w372) -> (s? t:f=w375:errorcluster)
            n197 = call <vilib>:"Simple Error Handler.vi"("error in (no error)"=w375) -> ()  [unwired: 4 in, 5 out]
          }
          frame Enabled {
          }
        }
        n198 = disable-structure shown="Disabled" {
          frame Disabled {
            n199 = call "VIH ExtCmd - Check VIHRUN Existence.vi"() -> ("Exist"=w366:bool)  [unwired: 7 in, 4 out]
            n200 = case shown="True" w366 {
              frame False {
              }
              frame True {
                n201 = call "VIH ExtCmd - Check VIHRUN Association.vi"() -> ("Associated"=w370:bool, "In LV Folder"=w368:bool)  [unwired: 7 in, 3 out]
                n202 = Not(x=w370) -> (.not. x?=w369:bool)
                n203 = And(x=w368, y=w369) -> (x .and. y?=w367:bool)
                n204 = case shown="True" w367 {
                  frame False {
                  }
                  frame True {
                    n205 = call "VIH ExtCmd - Associate VIHRUN.vi"() -> ()  [unwired: 11 in, 1 out]
                  }
                }
              }
            }
          }
          frame Enabled {
          }
        }
        n206 = Concatenate Strings("RW INI File = Read;\n\nEXTCMD = OPEN;\nINIT;\nEXTCMD = CHECK;\n\nOPEN FP = FORCE;\n\nQUICK TIPS;", w365) -> (w364:string)
      }
      frame "INIT" {
        n207 = control-ref of="Tree"() -> (w395:refnum<vi>)
        n208 = call "VIH Platform - Windows - Explore Folder.vi"("cmd (run)"=enum16{"run", "check"}."check") -> ("error out"=w386:errorcluster)  [unwired: 10 in]
        n209 = Unbundle By Name(w386) -> ("status"=w385:bool)
        n210 = call "VIH UI - Controller for Property Pages.vi"("cmd (update)"=T5."Open", "Project Tree"=w395) -> ("error out"=w393:errorcluster)  [unwired: 8 in, 1 out]
        n211 = Current VI's Menubar() -> (w389:refnum<k9>)
        n212 = Not(x=w385) -> (.not. x?=w384:bool)
        n213 = call "VIH Constant - Examples Folder.vi"() -> ("Examples folder"=w391:path)  [unwired: 11 in]
        n214 = Current VI's Menubar() -> (w392:refnum<k9>)
        n215 = call "VIH Utility - UI - Boolean to Control Disable Status.vi"("Status in"=w384) -> ("Control Disable if False"=w383:u8)  [unwired: 3 in, 1 out]
        n216 = Set Menu Item Info(7:"EXEC = Menu = Explore Build Root;" ("item tag"), 9:w384, 11:w389) -> ()  [unwired: 4 in, 2 out]
        n217 = call "VIH Project - Menu - Build Examples Menu.vi"("error in"=w393, "Examples folder"=w391, "menu reference"=w392) -> ()  [unwired: 7 in, 2 out]
        n218 = property on="%Toolbar_BuildExplore" class="Bool"("DisabledEnum"=w383) -> ()  [unwired: 2 in, 2 out]
        n219 = call "VIH Dialog - VI Terminals - Term Symbols.vi"("cmd (nop)"=T4."Init") -> ()  [unwired: 7 in, 4 out]
        n220 = Concatenate Strings("Project: New = Silent;", w398) -> (w397:string)
      }
      frame "OPEN FP" {
        n221 = call "VIH ExtCmd - Params Store.vi"() -> ("Params"=w405:T26)  [unwired: 10 in, 1 out]
        n222 = To Upper Case(1:w402) -> (0:w401:string)
        n223 = Unbundle By Name(w405) -> ("Show Window"=w404:bool)
        n224 = Equal?(x=w401, y="FORCE") -> (x = y?=w399:bool)
        n225 = Or(x=w399, y=w404) -> (x .or. y?=w403:bool)
        n226 = case shown="True" w403 {
          tunnel: w407 -> [_ w409]
          frame False {
          }
          frame True {
            n227 = invoke class="VI" method="FP.Open"(reference=w409, "Activate"=TRUE ("Activate?")) -> ()  [unwired: 3 in, 5 out]
          }
        }
      }
      frame "QUICK TIPS" {
        n228 = call "VIH HelpGen - Settings - Container.vi"() -> ("Settings out"=w411:T27)  [unwired: 10 in, 1 out]
        n229 = To Upper Case(1:w416) -> (0:w414:string)
        n230 = Unbundle By Name(w411) -> ("ShowQuickTips"=w412:bool, "NextQuickTip"=w410:i32)
        n231 = Equal?(x=w414, y="FORCE") -> (x = y?=w413:bool)
        n232 = Or(x=w413, y=w412) -> (x .or. y?=w417:bool)
        n233 = case shown="True" w417 {
          tunnel: w413 -> [_ w419]
          tunnel: w411 -> [_ w431]
          tunnel: w410 -> [_ w430]
          frame False {
          }
          frame True {
            n234 = First Call?() -> (First Call?: T/F=w422:bool)
            n235 = Not(x=w422) -> (.not. x?=w421:bool)
            n236 = And(x=w419, y=w421) -> (x .and. y?=w420:bool)
            n237 = Select(t=-1 ("Tip#"), s=w420, f=w430) -> (s? t:f=w433:i32)
            n238 = call "VIH Dialog - Quick Tips.vi"("Tip#"=w433) -> ("Tip# out"=w428:i32, "ShowAtStartup out"=w429:bool)  [unwired: 9 in]
            n239 = Increment(x=w428) -> (x+1=w426:i32)
            n240 = Bundle By Name(cluster=w431, "ShowQuickTips"=w429, "NextQuickTip"=w426) -> (w427:T27)
            n241 = call "VIH HelpGen - Settings - Container.vi"("cmd (get)"=enum16{"get", "set", "load", "save"}."set", "Settings in"=w427) -> ("error out"=w425:errorcluster)  [unwired: 8 in, 1 out]
            n242 = call "VIH HelpGen - Settings - Container.vi"("cmd (get)"=enum16{"get", "set", "load", "save"}."save", "error in"=w425) -> ()  [unwired: 8 in, 2 out]
          }
        }
      }
      frame "EXTCMD" {
        n243 = feedback #1() -> (w439:refnum<queue>)  [unwired: 1 in]
        n244 = case shown="\"CHECK\"" w441 {
          tunnel: [w443 w445 refnum<queue> refnum ("queue out") w452 w456] -> w440
          tunnel: w439 -> [w443 _ w450 w452 w456]
          tunnel: w438 -> [w442 _ _ _ _]
          tunnel: [_ _ _ _ w455] -> w434
          frame Default {
            n245 = One Button Dialog(message=w442) -> ()  [unwired: 1 in, 1 out]
          }
          frame "OPEN" {
            n246 = Obtain Queue(name (unnamed)="VIHelpeks Request Queue", element data type="") -> (queue out=w445:refnum<queue>)  [unwired: 3 in, 2 out]
            n247 = call "VIH ExtCmd - Params Store.vi"("cmd (get)"=enum16{"Init", "get", "set", "getcfg"}."Init") -> ()  [unwired: 9 in, 2 out]
          }
          frame "CLOSE" {
            n248 = Release Queue(queue=w450) -> ()  [unwired: 2 in, 3 out]
            n249 = call "VIH ExtCmd - Params Store.vi"("cmd (get)"=enum16{"Init", "get", "set", "getcfg"}."Init") -> ()  [unwired: 9 in, 2 out]
          }
          frame "RESET" {
            n250 = call "VIH ExtCmd - Params Store.vi"("cmd (get)"=enum16{"Init", "get", "set", "getcfg"}."Init") -> ()  [unwired: 9 in, 2 out]
          }
          frame "CHECK" {
            n251 = Dequeue Element(queue=w456, timeout in ms (-1)=0) -> (element=w454:string)  [unwired: 1 in, 3 out]
            n252 = Empty String/Path?(string/path=w454) -> (empty?=w453:bool)
            n253 = case shown="False" w453 {
              tunnel: w454 -> [w460 _]
              tunnel: [w458 _] -> w455
              frame False {
                n254 = while {
                  shift-right: [w461] -> _
                  shift-left: w460 -> [w467]
                  shift-right: [w464] -> w458
                  shift-left: "" -> [w463]
                  stop <- w462 stop-if-true
                  n255 = call "VIH Utility - APP - State Queue Parser (STR).vi"("input queue"=w467) -> ("state parameters"=w465:string, "state"=w466:string, "remained queue"=w461:string)  [unwired: 5 in, 1 out]
                  n256 = case shown="\"BUILD\"" w466 {
                    tunnel: w465 -> [_ w470 w486 _ _ w502 w511 w520 w529 w538]
                    tunnel: [w468 w472 w483 w493 w494 w503 w512 w521 w530 w539] -> w464
                    tunnel: w463 -> [w468 w474 w485 w491 w494 w503 w512 w521 w530 w539]
                    frame Default {
                    }
                    frame "OPEN" {
                      n257 = Empty String/Path?(string/path=w470) -> (empty?=w471:bool)
                      n258 = case shown="False" w471 {
                        tunnel: w470 -> [w477 _]
                        tunnel: [w475 ""] -> w473
                        frame False {
                          n259 = Format Into String(format string="OPEN FP = FORCE;\n\nAsk to Save Project;\n\nProject: New = Silent;\n\nSet Busy = ON;\nProject: Load XML = %s;\nSet Busy = OFF;", w477) -> (resulting string=w475:string)  [unwired: 2 in, 1 out]
                        }
                        frame True {
                        }
                      }
                      n260 = Concatenate Strings(w474, w473) -> (w472:string)
                      n261 = call "VIH ExtCmd - Params Store.vi"("cmd (get)"=enum16{"Init", "get", "set", "getcfg"}."Init") -> ()  [unwired: 9 in, 2 out]
                    }
                    frame "BUILD" {
                      (unwired) "EXEC = Menu = CHM Project;"
                      n262 = case shown="Default" w486 {
                        selector: w486 -> [_ w488]
                        tunnel: ["OPEN FP;\n\nEXEC = Project: Build = ALL;\n\nEXTCMD = RESET;" w489] -> w484
                        frame "", "CURRENT" {
                        }
                        frame Default {
                          n263 = Format Into String(format string="OPEN FP;\n\nAsk to Save Project;\n\nProject: New = Silent;\n\nSet Busy = ON;\nProject: Load XML = %s;\nSet Busy = OFF;\n\nEXEC = Project: Build = ALL;\n\nEXTCMD = RESET;", w488) -> (resulting string=w489:string)  [unwired: 2 in, 1 out]
                        }
                      }
                      n264 = call "VIH ExtCmd - Params Store.vi"("cmd (get)"=enum16{"Init", "get", "set", "getcfg"}."getcfg") -> ("Params"=w482:T26)  [unwired: 9 in, 1 out]
                      n265 = Concatenate Strings(w485, w484) -> (w483:string)
                      n266 = call "VIH ExtCmd - Params Store.vi"("cmd (get)"=enum16{"Init", "get", "set", "getcfg"}."set", "Params in"=w482, "Ext Command in"=TRUE) -> ()  [unwired: 7 in, 2 out]
                    }
                    frame "EXIT" {
                      n267 = Concatenate Strings(w491, "EXIT = EXTCMD;") -> (w493:string)
                    }
                    frame "---------------- 1" {
                    }
                    frame "OPT_ShowWindow" {
                      n268 = Scan From String(input string=w502, default 1=TRUE) -> (output 1=w497:bool)  [unwired: 3 in, 3 out]
                      n269 = call "VIH ExtCmd - Params Store.vi"("cmd (get)"=enum16{"Init", "get", "set", "getcfg"}."getcfg") -> ("Params"=w499:T26, "Ext Command"=w498:bool)  [unwired: 9 in]
                      n270 = Bundle By Name(cluster=w499, "Show Window"=w497) -> (w500:T26)
                      n271 = call "VIH ExtCmd - Params Store.vi"("cmd (get)"=enum16{"Init", "get", "set", "getcfg"}."set", "Params in"=w500, "Ext Command in"=w498) -> ()  [unwired: 7 in, 2 out]
                    }
                    frame "Opt_ShowProgress" {
                      n272 = Scan From String(input string=w511, default 1=TRUE) -> (output 1=w506:bool)  [unwired: 3 in, 3 out]
                      n273 = call "VIH ExtCmd - Params Store.vi"("cmd (get)"=enum16{"Init", "get", "set", "getcfg"}."getcfg") -> ("Params"=w508:T26, "Ext Command"=w507:bool)  [unwired: 9 in]
                      n274 = Bundle By Name(cluster=w508, "Show Progress"=w506) -> (w509:T26)
                      n275 = call "VIH ExtCmd - Params Store.vi"("cmd (get)"=enum16{"Init", "get", "set", "getcfg"}."set", "Params in"=w509, "Ext Command in"=w507) -> ()  [unwired: 7 in, 2 out]
                    }
                    frame "Opt_BuildHTML" {
                      n276 = Scan From String(input string=w520, default 1=TRUE) -> (output 1=w515:bool)  [unwired: 3 in, 3 out]
                      n277 = call "VIH ExtCmd - Params Store.vi"("cmd (get)"=enum16{"Init", "get", "set", "getcfg"}."getcfg") -> ("Params"=w517:T26, "Ext Command"=w516:bool)  [unwired: 9 in]
                      n278 = Bundle By Name(cluster=w517, "Generate HTML"=w515) -> (w518:T26)
                      n279 = call "VIH ExtCmd - Params Store.vi"("cmd (get)"=enum16{"Init", "get", "set", "getcfg"}."set", "Params in"=w518, "Ext Command in"=w516) -> ()  [unwired: 7 in, 2 out]
                    }
                    frame "Opt_BuildHHP" {
                      n280 = Scan From String(input string=w529, default 1=TRUE) -> (output 1=w524:bool)  [unwired: 3 in, 3 out]
                      n281 = call "VIH ExtCmd - Params Store.vi"("cmd (get)"=enum16{"Init", "get", "set", "getcfg"}."getcfg") -> ("Params"=w526:T26, "Ext Command"=w525:bool)  [unwired: 9 in]
                      n282 = Bundle By Name(cluster=w526, "Generate HHP"=w524) -> (w527:T26)
                      n283 = call "VIH ExtCmd - Params Store.vi"("cmd (get)"=enum16{"Init", "get", "set", "getcfg"}."set", "Params in"=w527, "Ext Command in"=w525) -> ()  [unwired: 7 in, 2 out]
                    }
                    frame "Opt_BuildCHM" {
                      n284 = Scan From String(input string=w538, default 1=TRUE) -> (output 1=w533:bool)  [unwired: 3 in, 3 out]
                      n285 = call "VIH ExtCmd - Params Store.vi"("cmd (get)"=enum16{"Init", "get", "set", "getcfg"}."getcfg") -> ("Params"=w535:T26, "Ext Command"=w534:bool)  [unwired: 9 in]
                      n286 = Bundle By Name(cluster=w535, "Generate CHM"=w533) -> (w536:T26)
                      n287 = call "VIH ExtCmd - Params Store.vi"("cmd (get)"=enum16{"Init", "get", "set", "getcfg"}."set", "Params in"=w536, "Ext Command in"=w534) -> ()  [unwired: 7 in, 2 out]
                    }
                  }
                  n288 = Empty String/Path?(string/path=w461) -> (empty?=w462:bool)
                }
              }
              frame True {
              }
            }
          }
        }
        n289 = feedback-in #1(w440) -> ()
        n290 = Empty String/Path?(string/path=w434) -> (empty?=w435:bool)
        n291 = Select(t=w436, s=w435, f=w434) -> (s? t:f=w437:string)
      }
      frame "EXIT" {
        n292 = Format Into String(format string="EXTCMD = CLOSE;\nKey Focus = Tree;\nHALT = %s;", w544) -> (resulting string=w546:string)  [unwired: 2 in, 1 out]
        n293 = case shown="Default" w544 {
          tunnel: [w548 w552 w555] -> w543
          tunnel: "Ask to Save Project;\n\nRW INI File = Write;" -> [w549 w554 _]
          tunnel: [w549 w554 _] -> w541
          tunnel: "Tree: New;" -> [w548 w553 w555]
          frame Default {
          }
          frame "KeepFPOpen" {
            n294 = Select(t=w553, s=TRUE, f="") -> (s? t:f=w552:string)
          }
          frame "EXTCMD" {
          }
        }
        n295 = Concatenate Strings(w541, w543, w546) -> (w545:string)
      }
      frame "HALT" {
        w557 = enum16{"get", "close"}."close" ("cmd (get)")
        n296 = control-ref of="Tree"() -> (w567:refnum<vi>)
        n297 = control-ref of="Sub Panel"() -> (w565:refnum<vi>)
        n298 = call "VIH UI - Controller for Property Pages.vi"("cmd (update)"=T5."Close", "SubPanel"=w565, "Project Tree"=w567) -> ("error out"=w564:errorcluster)  [unwired: 7 in, 1 out]
        n299 = call "VIH HelpGen - Open VI Reference - Temp VI Refnum.vi"("cmd (get)"=w557) -> ("error out"=w561:errorcluster)  [unwired: 9 in, 1 out]
        n300 = call "VIH HelpGen - Get Control Terminal Image - Temp VI Refnum.vi"("cmd (get)"=w557, "error in"=w561) -> ("error out"=w556:errorcluster)  [unwired: 8 in, 1 out]
        n301 = property class="VI"(reference=w560, error in=w564, "Front Panel.Title"=w570) -> (reference out=w559:refnum<vi>, error out=w568:errorcluster)
        n302 = call "VIH Constant - Temporal Build Log File.vi"() -> ("Temporal Build Log File"=w563:path)  [unwired: 11 in]
        n303 = call "VIH ProjFile - Core.vi"("cmd (get)"=enum16{"get", "create", "load", "save", "close"}."close", "error in"=w568) -> ("error out"=w569:errorcluster)  [unwired: 8 in, 1 out]
        n304 = Delete(path (use dialog)=w563, error in=w556) -> (error out=w562:errorcluster)  [unwired: 3 in, 2 out]
        n305 = case shown="\"EXTCMD\"" w572 {
          tunnel: w569 -> [_ _ _]
          tunnel: w562 -> [_ _ _]
          tunnel: w559 -> [w576 w578 w582]
          tunnel: [w575 w577 w582] -> w558
          frame Default {
            n306 = invoke class="VI" method="FP.Close"(reference=w576) -> (reference out=w575:refnum<vi>)  [unwired: 2 in, 2 out]
          }
          frame "EXTCMD" {
            n307 = disable-structure shown="Disabled" {
              disable-tunnel: w578 -> [w580 w581]
              disable-tunnel: [w579 w581] -> w577
              frame Disabled {
                n308 = invoke class="VI" method="FP.Close"(reference=w580) -> (reference out=w579:refnum<vi>)  [unwired: 2 in, 2 out]
              }
              frame Enabled {
              }
            }
          }
          frame "KeepFPOpen" {
          }
        }
        n309 = Close Reference(reference=w558) -> ()  [unwired: 1 in, 1 out]
      }
      frame "------------------------------- 1" {
      }
      frame "RW INI File" {
        n310 = call "VIH Constant - Main INI File.vi"() -> ("Main INI File"=w584:path, "Section"=w588:string)  [unwired: 10 in]
        n311 = case shown="\"Write\"" w597 {
          tunnel: [enum16{"read", "write"}."read" ("cmd (read)") enum16{"read", "write"}."write" ("cmd (read)") _] -> w592
          tunnel: [enum16{"get", "set", "load", "save"}."load" ("cmd (get)") enum16{"get", "set", "load", "save"}."save" ("cmd (get)") _] -> w587
          tunnel: w584 -> [_ w603 _]
          frame "Read" {
          }
          frame "Write" {
            n312 = Strip Path(path=w603) -> (stripped path=w602:path)  [unwired: 1 out]
            n313 = File/Directory Info(path=w602) -> (error out=w601:errorcluster)  [unwired: 1 in, 6 out]
            n314 = case shown="Error" w601 {
              tunnel: w602 -> [_ w606]
              frame No Error {
              }
              frame Error {
                n315 = Create Folder(path (use dialog)=w606) -> ()  [unwired: 2 in, 3 out]
              }
            }
          }
          frame Default {
            n316 = call <vilib>:"Beep.vi"() -> ()  [unwired: 12 in]
          }
        }
        n317 = call <vilib>:"Open Config Data.vi"("configuration file path"=w584) -> ("error out"=w594:errorcluster, "refnum"=w596:T28)  [unwired: 8 in, 1 out]
        n318 = Build Array("RecentProjects" ("menu tag")) -> (w590:string[])
        n319 = Current VI's Menubar() -> (w591:refnum<k9>)
        n320 = call "VIH Utility - MENU - Recent Paths - RW INI File.vi"("cmd (read)"=w592, "section"=w588, "error in"=w594, "Menu Tags"=w590, "Menu Refnum"=w591, "INI refnum"=w596) -> ("error out"=w593:errorcluster, "dup INI refnum"=w595:T28)  [unwired: 4 in]
        n321 = call <vilib>:"Close Config Data.vi"("error in (no error)"=w593, "refnum"=w595) -> ("error out"=w585:errorcluster)  [unwired: 8 in, 1 out]
        n322 = call <vilib>:"Clear Errors.vi"("error in (no error)"=w585) -> ("error out"=w586:errorcluster)  [unwired: 5 in, 1 out]
        n323 = call "VIH HelpGen - Settings - Container.vi"("cmd (get)"=w587, "error in"=w586) -> ()  [unwired: 8 in, 2 out]
      }
      frame "Set Busy" {
        n324 = case shown="\"ON\"" w607 {
          frame Default {
            n325 = call <vilib>:"Unset Busy.vi"() -> ()  [unwired: 11 in, 1 out]
          }
          frame "ON" {
            n326 = call <vilib>:"Set Busy.vi"() -> ()  [unwired: 10 in, 2 out]
          }
        }
      }
      frame "Defer FP Update" {
        n327 = To Upper Case(1:w612) -> (0:w611:string)
        n328 = Equal?(x=w611, y="ON") -> (x = y?=w609:bool)
        n329 = property class="VI"() -> ("Panel"=w613:refnum<vi>)  [unwired: 2 in, 2 out]
        n330 = property class="Pnl"(reference=w613, "DeferPanUpdts"=w609) -> ()  [unwired: 1 in, 2 out]
      }
      frame "Key Focus" {
        n331 = case shown="\"Tree\"" w615 {
          frame Default {
          }
          frame "Tree" {
            n332 = control-ref of="Tree"() -> (w617:refnum<vi>)
            n333 = call "VIH Utility - UI - Key Focus & Selection Color (Tree Control).vi"("F:Test/T:Set Key Focus (F)"=TRUE ("Key Focus"), "Tree Refnum"=w617) -> ()  [unwired: 7 in, 3 out]
          }
        }
      }
      frame "Menu" {
        n334 = control-ref of="Tree"() -> (w621:refnum<vi>)
        n335 = Match Pattern(string=w629, regular expression="\\?") -> (before substring=w627:string, after substring=w626:string)  [unwired: 1 in, 2 out]
        n336 = call <vilib>:"Trim Whitespace.vi"("string"=w627) -> ("trimmed string"=w625:string)  [unwired: 1 in]
        n337 = call <vilib>:"Trim Whitespace.vi"("string"=w626) -> ("trimmed string"=w620:string)  [unwired: 1 in]
        n338 = case shown="\"CHM Project\"" w625 {
          tunnel: w624 -> [w632 _ _ _ _ _ _ _ _ _ _ _ _ _ _ _ _ _ _ _ _ _ _ _ _ _ _]
          tunnel: ["" w634 w664 w712 _ _ _ _ _ _ _ _ w883 _ w910 "Defer FP Update = ON;\nUpdate Controls;\nDefer FP Update = OFF;" ("format string") w962 _ w991 _ "Update Window Title;\nUpdate Toolbar;" ("format string") "Update Toolbar;" _ _ _ _ _] -> w622
          tunnel: w621 -> [_ w633 w665 w713 _ _ _ _ _ w853 _ _ _ _ w909 w947 w961 w978 w990 _ w1010 _ _ _ _ _ _]
          tunnel: w620 -> [_ _ w663 w711 _ _ _ _ _ _ _ _ _ _ w911 _ _ _ _ _ _ w1014 _ _ _ _ _]
          tunnel: w619 -> [_ _ _ _ _ w750 w796 w839 w850 w852 _ _ _ _ w906 w945 _ _ w987 _ _ w1022 _ _ _ _ _]
          frame Default {
            n339 = One Button Dialog(message=w632) -> ()  [unwired: 1 in, 1 out]
          }
          frame "WARNING" {
            n340 = call "VIH Project Tree - Find Invalid Files in Project Tree.vi"("Project Tree"=w633) -> ("Item Paths"=w638:path[], "dup Project Tree"=w639:T24)  [unwired: 7 in, 2 out]
            n341 = Empty Array?(array=w638) -> (empty?=w637:bool)
            n342 = case shown="True" w637 {
              tunnel: w639 -> [_ w645]
              tunnel: [w640 w644] -> w634
              tunnel: "Menu = Rule List ? Lost;" -> [_ w643]
              tunnel: "Menu = File List ? Invalid;" -> [w640 _]
              frame False {
              }
              frame True {
                n343 = call "VIH Project - Verify CSS,JS,Template Files.vi"() -> ("error"=w642:bool, "Message"=w641:string)  [unwired: 9 in, 1 out]
                n344 = case shown="False" w642 {
                  tunnel: w645 -> [w651 _]
                  tunnel: [w648 _] -> w644
                  tunnel: w643 -> [w646 _]
                  tunnel: w641 -> [_ w652]
                  frame False {
                    n345 = call "VIH Project Tree - Find Lost Item Rules.vi"("Project Tree"=w651) -> ("Lost Rules (Owner Paths)"=w650:path[])  [unwired: 8 in, 2 out]
                    n346 = Empty Array?(array=w650) -> (empty?=w649:bool)
                    n347 = Select(t="", s=w649, f=w646) -> (s? t:f=w648:string)
                  }
                  frame True {
                    n348 = One Button Dialog(message=w652) -> ()  [unwired: 1 in, 1 out]
                  }
                }
              }
            }
          }
          frame "File List" {
            n349 = To Lower Case(string=w663) -> (all lower case string=w662:string)
            n350 = Equal?(x=w662, y="invalid") -> (x = y?=w654:bool)
            n351 = Select(t=enum32{"ALL", "conpane", "invalid"}."invalid" ("File set (All)"), s=w654, f=enum32{"ALL", "conpane", "invalid"}."ALL" ("File set (All)")) -> (s? t:f=w655:enum32{"ALL", "conpane", "invalid"})
            n352 = call "VIH Dialog - Project File List.vi"("File set (All)"=w655, "Called from Master (F)"=TRUE, "Project Tree"=w665) -> ("OK out"=w659:bool, "File Paths"=w666:path[])  [unwired: 6 in, 1 out]
            n353 = Empty Array?(array=w666) -> (empty?=w660:bool)
            n354 = Compound Arithmetic op=AND(invert w660, w659) -> (w658:bool)
            n355 = case shown="True" w658 {
              tunnel: w666 -> [_ w673]
              tunnel: ["Set Busy = ON;\nDefer FP Update = ON;\n\nUpdate Toolbar: Warning;\n\nDefer FP Update = OFF;\nSet Busy = OFF;\n\nKey Focus = Tree;" ("format string") "Set Busy = ON;\nDefer FP Update = ON;\n\nUpdate Controls;\nUpdate Toolbar: Warning;\n\nDefer FP Update = OFF;\nSet Busy = OFF;\n\nKey Focus = Tree;" ("format string")] -> w664
              frame False {
              }
              frame True {
                w671 = string[] []
                # "put Static instances to the end"
                n356 = property on="Tree" class="Tree (strict)"() -> ("All Tags"=w674:string[])  [unwired: 2 in, 2 out]
                n357 = for {
                  tunnel: w674 -> [w682] mode=indexing
                  shift-right: [w683] -> w670
                  shift-left: w671 -> [w684]
                  tunnel: w673 -> [w681]
                  shift-right: [w679] -> w669
                  shift-left: w671 -> [w680]
                  n358 = call "VIH Project Tree - Item Tag - Parse.vi"("Tree Item Tag"=w682) -> ("Item File Path"=w685:path, "Item Type"=w677:T2)  [unwired: 8 in, 1 out]
                  n359 = call "VIH Project Tree - Item Type to Boolean Flags.vi"("Item Type"=w677) -> ("Dynamic"=w676:bool)  [unwired: 4 in, 6 out]
                  n360 = Search 1D Array(1D array=w681, element=w685) -> (index of element=w678:i32)  [unwired: 1 in]
                  n361 = case shown="0.." w678 {
                    tunnel: w684 -> [w687 w693]
                    tunnel: [w687 w692] -> w683
                    tunnel: w682 -> [_ w691]
                    tunnel: w680 -> [w686 w690]
                    tunnel: [w686 w689] -> w679
                    tunnel: w676 -> [_ w688]
                    frame ..-1 {
                    }
                    frame 0.. {
                      n362 = case shown="False" w688 {
                        tunnel: w693 -> [w695 w701]
                        tunnel: [w695 w700] -> w692
                        tunnel: w691 -> [w694 w699]
                        tunnel: w690 -> [w697 w698]
                        tunnel: [w696 w698] -> w689
                        frame False {
                          n363 = Build Array (concatenate)(w697, w694) -> (w696:string[])
                        }
                        frame True {
                          n364 = Build Array (concatenate)(w701, w699) -> (w700:string[])
                        }
                      }
                    }
                  }
                }
                n365 = Build Array (concatenate)(w670, w669) -> (w668:string[])
                n366 = property on="Tree" class="Tree (strict)"("Value"=w668) -> ()  [unwired: 2 in, 2 out]
                n367 = for {
                  tunnel: w668 -> [w675] mode=indexing
                  n368 = invoke on="Tree" class="Tree (strict)" method="Open/Close.Ensure Visible"("tag"=w675) -> ()  [unwired: 3 in, 4 out]
                }
              }
            }
          }
          frame "Rule List" {
            n369 = To Lower Case(string=w711) -> (all lower case string=w710:string)
            n370 = Equal?(x=w710, y="lost") -> (x = y?=w705:bool)
            n371 = Select(t=enum32{"ALL", "lost"}."lost", s=w705, f=enum32{"ALL", "lost"}."ALL" ("File set (All)")) -> (s? t:f=w702:enum32{"ALL", "lost"})
            n372 = call "VIH Dialog - Project File Rules.vi"("File set (All)"=w702, "Project Tree"=w713) -> ("OK out"=w707:bool, "File Paths"=w714:path[])  [unwired: 8 in]
            n373 = Empty Array?(array=w714) -> (empty?=w708:bool)
            n374 = Compound Arithmetic op=AND(invert w708, w707) -> (w706:bool)
            n375 = case shown="True" w706 {
              tunnel: w714 -> [_ w721]
              tunnel: ["Set Busy = ON;\nDefer FP Update = ON;\n\nUpdate Controls;\nUpdate Toolbar: Warning;\n\nDefer FP Update = OFF;\nSet Busy = OFF;\n\nKey Focus = Tree;" ("format string") "Set Busy = ON;\nDefer FP Update = ON;\n\nUpdate Controls;\nUpdate Toolbar: Warning;\n\nDefer FP Update = OFF;\nSet Busy = OFF;\n\nKey Focus = Tree;" ("format string")] -> w712
              frame False {
                (unwired) "Key Focus = Tree;" ("format string")
              }
              frame True {
                w719 = string[] []
                # "put Static instances to the end"
                n376 = property on="Tree" class="Tree (strict)"() -> ("All Tags"=w722:string[])  [unwired: 2 in, 2 out]
                n377 = for {
                  tunnel: w722 -> [w730] mode=indexing
                  shift-right: [w731] -> w718
                  shift-left: w719 -> [w732]
                  tunnel: w721 -> [w729]
                  shift-right: [w727] -> w717
                  shift-left: w719 -> [w728]
                  n378 = call "VIH Project Tree - Item Tag - Parse.vi"("Tree Item Tag"=w730) -> ("Item File Path"=w733:path, "Item Type"=w725:T2)  [unwired: 8 in, 1 out]
                  n379 = call "VIH Project Tree - Item Type to Boolean Flags.vi"("Item Type"=w725) -> ("Dynamic"=w724:bool)  [unwired: 4 in, 6 out]
                  n380 = Search 1D Array(1D array=w729, element=w733) -> (index of element=w726:i32)  [unwired: 1 in]
                  n381 = case shown="0.." w726 {
                    tunnel: w732 -> [w735 w741]
                    tunnel: [w735 w740] -> w731
                    tunnel: w730 -> [_ w739]
                    tunnel: w728 -> [w734 w738]
                    tunnel: [w734 w737] -> w727
                    tunnel: w724 -> [_ w736]
                    frame ..-1 {
                    }
                    frame 0.. {
                      n382 = case shown="False" w736 {
                        tunnel: w741 -> [w743 w749]
                        tunnel: [w743 w748] -> w740
                        tunnel: w739 -> [w742 w747]
                        tunnel: w738 -> [w745 w746]
                        tunnel: [w744 w746] -> w737
                        frame False {
                          n383 = Build Array (concatenate)(w745, w742) -> (w744:string[])
                        }
                        frame True {
                          n384 = Build Array (concatenate)(w749, w747) -> (w748:string[])
                        }
                      }
                    }
                  }
                }
                n385 = Build Array (concatenate)(w718, w717) -> (w716:string[])
                n386 = property on="Tree" class="Tree (strict)"("Value"=w716) -> ()  [unwired: 2 in, 2 out]
                n387 = for {
                  tunnel: w716 -> [w723] mode=indexing
                  n388 = invoke on="Tree" class="Tree (strict)" method="Open/Close.Ensure Visible"("tag"=w723) -> ()  [unwired: 3 in, 4 out]
                }
              }
            }
          }
          frame "----------------------------- 1" {
          }
          frame "Open Source File" {
            (unwired) VIH_Project_Tree_Typedef_-_Tree_Item_Type."<Invalid>" ("Item Type")
            n389 = Index Array(array=w750) -> (element=w753:string)  [unwired: 1 in]
            n390 = call "VIH Project Tree - Item Tag - Parse.vi"("Tree Item Tag"=w753) -> ("Item File Path"=w754:path, "Item Type"=w752:T2)  [unwired: 8 in, 1 out]
            n391 = case shown="\"Any File\"" w752 {
              tunnel: w754 -> [_ w757 w777 w788]
              tunnel: [_ w758 w776 w789] -> w751
              frame Default {
                n392 = call <vilib>:"Beep.vi"() -> ()  [unwired: 12 in]
              }
              frame "Any File" {
                n393 = call "VIH Platform - Windows - Shell Execute.vi"("Shell action (open)"=T6."open", "exe/doc/dir path"=w757) -> ("error out"=w756:errorcluster)  [unwired: 9 in]
                n394 = case shown="No Error" w756 {
                  selector: w756 -> [w759 _]
                  tunnel: [w759 w761] -> w758
                  tunnel: w757 -> [_ w760]
                  frame No Error {
                  }
                  frame Error {
                    n395 = call-poly <vilib>:"Open URL in Default Browser.vi"("path"=w760) -> ("error out"=w761:errorcluster)  [unwired: 5 in, 1 out]
                  }
                }
              }
              frame ".vi".."expVI (dyn)", "PolyVI Inst" {
                (unwired) 2 ("options")
                n396 = Open VI Reference(vi path=w777, options=0) -> (vi reference=w766:refnum<vi>, error out=w773:errorcluster)  [unwired: 4 in]
                n397 = property class="VI"(reference=w766, error in=w773) -> ("FP.Behavior"=w770:T8, "Exec.State"=w772:T7)  [unwired: 2 out]
                n398 = Greater?(x=w772, y=T7."Idle" ("Execution:State")) -> (0:w767:bool)
                n399 = Equal?(x=T8."Modal" ("y"), y=w770) -> (x = y?=w768:bool)
                n400 = And(x=w768, y=w767) -> (x .and. y?=w764:bool)
                n401 = case shown="True" w764 {
                  tunnel: [TRUE w780] -> w765
                  tunnel: "The VI belongs to a running hierarchy and it's Front Panel is Modal.\n\nAre you sure to open the VI?" -> [_ w779]
                  frame False {
                  }
                  frame True {
                    n402 = Two Button Dialog(message=w779) -> (T button?=w780:bool)  [unwired: 2 in]
                  }
                }
                n403 = case shown="True" w765 {
                  tunnel: [w782 w787] -> w775
                  tunnel: [w781 w786] -> w774
                  tunnel: w773 -> [w782 w784]
                  tunnel: w766 -> [w781 w783]
                  frame False {
                  }
                  frame True {
                    n404 = invoke class="VI" method="FP.Open"(reference=w783, error in=w784, "Activate"=TRUE ("Activate?")) -> (reference out=w786:refnum<vi>, error out=w787:errorcluster)  [unwired: 2 in, 3 out]
                  }
                }
                n405 = Close Reference(reference=w774, error in (no error)=w775) -> (error out=w776:errorcluster)
              }
              frame "HTML" {
                n406 = call-poly <vilib>:"Open URL in Default Browser.vi"("path"=w788) -> ("error out"=w789:errorcluster)  [unwired: 5 in, 1 out]
              }
            }
            n407 = call <vilib>:"Simple Error Handler.vi"("error in (no error)"=w751) -> ()  [unwired: 4 in, 5 out]
          }
          frame "Edit Source File" {
            (unwired) VIH_Project_Tree_Typedef_-_Tree_Item_Type."<Invalid>" ("Item Type")
            n408 = call "VIH HelpGen - Settings - Container.vi"() -> ("Settings out"=w793:T27)  [unwired: 10 in, 1 out]
            n409 = Index Array(array=w796) -> (element=w799:string)  [unwired: 1 in]
            n410 = Unbundle By Name(w793) -> ("EditPrgs"=w792:T29)
            n411 = call "VIH Project Tree - Item Tag - Parse.vi"("Tree Item Tag"=w799) -> ("Item File Path"=w795:path, "Item Type"=w798:T2)  [unwired: 8 in, 1 out]
            n412 = call "VIH HelpGen - Settings - Get Program for File Type.vi"("EditPrograms"=w792, "File Path"=w795) -> ("Found"=w791:bool, "Program Path"=w790:path, "dup File Path"=w794:path)  [unwired: 7 in]
            n413 = case shown="False" w791 {
              tunnel: w798 -> [w802 _]
              tunnel: [w801 w836] -> w797
              tunnel: w794 -> [w800 w832]
              tunnel: w790 -> [_ w837]
              frame False {
                n414 = case shown="\"Any File\", \"HTML\"" w802 {
                  tunnel: w800 -> [_ w805 w821]
                  tunnel: [_ w803 w820] -> w801
                  frame Default {
                    n415 = call <vilib>:"Beep.vi"() -> ()  [unwired: 12 in]
                  }
                  frame "Any File", "HTML" {
                    n416 = call "VIH Platform - Windows - Shell Execute.vi"("Shell action (open)"=T6."edit", "exe/doc/dir path"=w805) -> ("error out"=w803:errorcluster)  [unwired: 9 in]
                  }
                  frame ".vi".."expVI (dyn)", "PolyVI Inst" {
                    n417 = Open VI Reference(vi path=w821, options=2) -> (vi reference=w810:refnum<vi>, error out=w817:errorcluster)  [unwired: 4 in]
                    n418 = property class="VI"(reference=w810, error in=w817) -> ("FP.Behavior"=w814:T8, "Exec.State"=w816:T7)  [unwired: 2 out]
                    n419 = Greater?(x=w816, y=T7."Idle" ("Execution:State")) -> (0:w811:bool)
                    n420 = Equal?(x=T8."Modal" ("y"), y=w814) -> (x = y?=w812:bool)
                    n421 = And(x=w812, y=w811) -> (x .and. y?=w808:bool)
                    n422 = case shown="True" w808 {
                      tunnel: [TRUE w824] -> w809
                      tunnel: "The VI belongs to a running hierarchy and it's Front Panel is Modal.\n\nAre you sure to open the VI?" -> [_ w823]
                      frame False {
                      }
                      frame True {
                        n423 = Two Button Dialog(message=w823) -> (T button?=w824:bool)  [unwired: 2 in]
                      }
                    }
                    n424 = case shown="True" w809 {
                      tunnel: [w826 w831] -> w819
                      tunnel: [w825 w830] -> w818
                      tunnel: w817 -> [w826 w828]
                      tunnel: w810 -> [w825 w827]
                      frame False {
                      }
                      frame True {
                        n425 = invoke class="VI" method="FP.Open"(reference=w827, error in=w828, "Activate"=TRUE ("Activate?")) -> (reference out=w830:refnum<vi>, error out=w831:errorcluster)  [unwired: 2 in, 3 out]
                      }
                    }
                    n426 = Close Reference(reference=w818, error in (no error)=w819) -> (error out=w820:errorcluster)
                  }
                }
              }
              frame True {
                n427 = Format Into String(format string="\"%s\" \"%s\"", w837, w832) -> (resulting string=w834:string)  [unwired: 2 in, 1 out]
                n428 = call <vilib>:"System Exec.vi"("wait until completion? (T)"=FALSE, "command line"=w834) -> ("error out"=w836:errorcluster)  [unwired: 6 in, 3 out]
              }
            }
            n429 = call <vilib>:"Simple Error Handler.vi"("error in (no error)"=w797) -> ()  [unwired: 4 in, 5 out]
          }
          frame "VI Terminals" {
            n430 = Index Array(array=w839) -> (element=w840:string)  [unwired: 1 in]
            n431 = call "VIH Project Tree - Item Tag - Parse.vi"("Tree Item Tag"=w840) -> ("Item File Path"=w841:path)  [unwired: 8 in, 2 out]
            n432 = call "VIH Dialog - VI Terminals.vi"("Called from Master (F)"=TRUE, "VI Path"=w841) -> ()  [unwired: 6 in, 4 out]
          }
          frame "VI Documentation" {
            # "dynamic call VI Doc Editor.vi\n\nThis way it's possible to start the Doc Editor from the Tools menu when VI Helpeks GUI is running"
            n433 = Index Array(array=w850) -> (element=w851:string)  [unwired: 1 in]
            n434 = call "VIH Project Tree - Item Tag - Parse.vi"("Tree Item Tag"=w851) -> ("Item File Path"=w842:path)  [unwired: 8 in, 2 out]
            n435 = vi-ref "VI Doc Editor.vi"() -> (w849:refnum<vi>)
            n436 = property class="VI"(reference=w849) -> ("Path"=w848:path)  [unwired: 1 in, 2 out]
            n437 = Open VI Reference(type specifier VI Refnum (for type only)=refnum<vi> refnum, vi path=w848) -> (vi reference=w845:refnum<vi>, error out=w846:errorcluster)  [unwired: 4 in]
            n438 = call-by-ref "?"(reference=w845, error in=w846, "VI Path in"=w842) -> (reference out=w844:refnum<vi>, error out=w843:errorcluster)  [unwired: 9 in, 2 out]
            n439 = Close Reference(reference=w844, error in (no error)=w843) -> ()  [unwired: 1 out]
          }
          frame "Open Output Help" {
            n440 = Index Array(array=w852) -> (element=w856:string)  [unwired: 1 in]
            n441 = call "VIH Project Tree - Item Tag - Parse.vi"("Tree Item Tag"=w856) -> ("Item File Path"=w864:path, "Item Type"=w862:T2)  [unwired: 8 in, 1 out]
            n442 = call "VIH Project - Get Effective File Rule.vi"("Ignore Control Rules (F)"=TRUE, "File Path"=w864, "Project Tree"=w853) -> ("Effective File Rule"=w854:T30)  [unwired: 5 in, 3 out]
            n443 = call "VIH Project Tree - Item Type to Palette Item Type.vi"("Tree Item Type"=w862) -> ("Item/File Type"=w863:T33)  [unwired: 9 in, 1 out]
            n444 = Unbundle By Name(w854) -> ("Target Paths.HTML Dir"=w858:path, "OutName"=w857:string)
            n445 = call "VIH HelpGen - Get Target HTML Filename.vi"("Item File Path"=w864, "Item Type"=w863, "HTML Filename in"=w857) -> ("HTML Fileame out"=w859:string)  [unwired: 7 in, 1 out]
            n446 = Build Path(base path=w858, name or relative path=w859) -> (appended path=w860:path)
            n447 = call-poly <vilib>:"Open URL in Default Browser.vi"("path"=w860) -> ("error out"=w861:errorcluster)  [unwired: 5 in, 1 out]
            n448 = call <vilib>:"Simple Error Handler.vi"("error in (no error)"=w861) -> ()  [unwired: 4 in, 5 out]
          }
          frame "Open Build Log" {
            n449 = call "VIH Project - Container - Project File Path.vi"() -> ("Project Build Log File"=w867:path)  [unwired: 9 in, 2 out]
            n450 = call "VIH UI - Test Path.vi"("Path"=w867) -> ("Good Path"=w866:bool, "dup Path"=w865:path)  [unwired: 7 in, 2 out]
            n451 = case shown="True" w866 {
              tunnel: w865 -> [_ w868]
              frame False {
              }
              frame True {
                n452 = call-poly <vilib>:"Open URL in Default Browser.vi"("path"=w868) -> ()  [unwired: 5 in, 2 out]
              }
            }
          }
          frame "Explore Build Root" {
            n453 = call "VIH Project - Container - Master Rule.vi"() -> ("Rule out"=w873:T15)  [unwired: 11 in]
            n454 = Unbundle By Name(w873) -> ("Build Root Dir"=w872:path)
            n455 = while {
              tunnel: [w877] -> w871
              shift-right: [w880] -> _
              shift-left: w872 -> [w882]
              stop <- w874 stop-if-true
              n456 = call "VIH UI - Test Path.vi"("Folder (F)"=TRUE, "Path"=w882) -> ("Good Path"=w876:bool, "dup Path"=w877:path)  [unwired: 6 in, 2 out]
              n457 = Empty String/Path?(string/path=w877) -> (empty?=w879:bool)
              n458 = Not A Number/Path/Refnum?(number/path/refnum=w877) -> (NaN/Path/Refnum?=w878:bool)
              n459 = Strip Path(path=w877) -> (stripped path=w880:path)  [unwired: 1 out]
              n460 = Or(x=w879, y=w878) -> (x .or. y?=w875:bool)
              n461 = Or(x=w876, y=w875) -> (x .or. y?=w874:bool)
            }
            n462 = call "VIH Platform - Windows - Explore Folder.vi"("cmd (run)"=enum16{"run", "check"}."run", "exe/doc/dir path"=w871) -> ("error out"=w869:errorcluster)  [unwired: 9 in]
            n463 = call <vilib>:"Simple Error Handler.vi"("error in (no error)"=w869) -> ()  [unwired: 4 in, 5 out]
          }
          frame "Cleanup Build Folder" {
            n464 = call "VIH Project - Container - Master Rule.vi"() -> ("Rule out"=w888:T15)  [unwired: 11 in]
            n465 = Unbundle By Name(w888) -> ("Build Root Dir"=w884:path)
            n466 = Format Into String(format string="Delete all files and folders in the Build Root Folder:\n%s\n\nAre you sure?", w884) -> (resulting string=w886:string)  [unwired: 2 in, 1 out]
            n467 = Two Button Dialog(message=w886) -> (T button?=w885:bool)  [unwired: 2 in]
            n468 = case shown="True" w885 {
              tunnel: w884 -> [_ w897]
              tunnel: [_ "Update Toolbar;"] -> w883
              frame False {
              }
              frame True {
                n469 = List Folder(path=w897) -> (path out=w894:path, filenames=w896:string[], folder names=w895:string[])  [unwired: 3 in, 1 out]
                n470 = Build Array (concatenate)(w896, w895) -> (w893:string[])
                n471 = for {
                  tunnel: w894 -> [w904]
                  tunnel: w893 -> [w903] mode=indexing
                  shift-right: [w899] -> w892
                  shift-left: errorcluster {"status"=FALSE, "code"=0, "source"=""} ("error IO") -> [w900]
                  n472 = Build Path(base path=w904, name or relative path=w903) -> (appended path=w902:path)
                  n473 = Delete(path (use dialog)=w902, entire hierarchy (F)=TRUE) -> (error out=w898:errorcluster)  [unwired: 3 in, 2 out]
                  n474 = Merge Errors(w900, w898) -> (w899:errorcluster)
                }
                n475 = call "VIH HelpGen - FILE - Check File Path (Buffered).vi"("cmd (get)"=enum16{"Init", "get"}."Init") -> ()  [unwired: 9 in, 2 out]
                n476 = call <vilib>:"Simple Error Handler.vi"("error in (no error)"=w892) -> ()  [unwired: 4 in, 5 out]
              }
            }
          }
          frame "----------------------------- 2" {
          }
          frame "Add File" {
            n477 = Index Array(array=w906) -> (element=w907:string)  [unwired: 1 in]
            n478 = case shown="\"Menu\"" w911 {
              tunnel: ["*.*" "*.mnu" "*.vi;*.vit" "*.html;*.htm"] -> w913
              frame "Misc", Default {
              }
              frame "Menu" {
              }
              frame "VI" {
              }
              frame "HTML" {
              }
            }
            n479 = call "VIH Project Tree - Find Group to Add Item.vi"("Item Tag"=w907, "Project Tree"=w909) -> ("Item Tag (Group)"=w905:string, "dup Project Tree"=w908:T24)  [unwired: 7 in, 1 out]
            n480 = call "File Dialog2"("prompt"="Add file(s) to project", "pattern (all files)"=w913) -> ("selected paths"=w915:path[], "error out"=w914:errorcluster)  [unwired: 10 in, 2 out]
            n481 = case shown="No Error" w914 {
              tunnel: w908 -> [w926 _]
              tunnel: w915 -> [w927 _]
              tunnel: ["Defer FP Update = ON;\nUpdate Controls;\nDefer FP Update = OFF;" ("format string") _] -> w910
              tunnel: w905 -> [w920 _]
              frame No Error {
                n482 = call "VIH Project Tree - Add Files.vi"("Ena dialog message (F)"=TRUE, "File Paths"=w927, "Tree Parent Tag"=w920, "Project Tree"=w926) -> ("error out"=w928:errorcluster, "Top-level Item Tags"=w924:string[], "dup Project Tree"=w922:T24)  [unwired: 4 in, 1 out]
                n483 = Empty Array?(array=w924) -> (empty?=w923:bool)
                n484 = case shown="False" w923 {
                  tunnel: w928 -> [w932 _]
                  tunnel: w924 -> [w931 _]
                  tunnel: w922 -> [w933 _]
                  frame False {
                    n485 = call "VIH Project Tree - Create Unique Output Names for Added Files.vi"("error in"=w932, "Added Item Tags"=w931, "Project Tree"=w933) -> ("error out"=w930:errorcluster, "dup Project Tree"=w929:T24)  [unwired: 7 in]
                    n486 = property class="Tree (strict)"(reference=w929, error in=w930, "Value"=w931) -> (reference out=w936:T24, error out=w934:errorcluster)
                    n487 = Index Array(array=w931) -> (element=w935:string)  [unwired: 1 in]
                    n488 = invoke class="Tree (strict)" method="Open/Close.Ensure Visible"(reference=w936, error in=w934, "tag"=w935) -> ()  [unwired: 1 in, 4 out]
                  }
                  frame True {
                  }
                }
              }
              frame Error {
              }
            }
          }
          frame "Add Group" {
            n489 = Index Array(array=w945) -> (element=w944:string)  [unwired: 1 in]
            n490 = call "VIH Project Tree - Find Group to Add Item.vi"("Item Tag"=w944, "Project Tree"=w947) -> ("Item Tag (Group)"=w943:string, "dup Project Tree"=w946:T24)  [unwired: 7 in, 1 out]
            n491 = call "VIH Project Tree - Add File Group.vi"("Tree Parent Tag"=w943, "Project Tree"=w946) -> ("error out"=w940:errorcluster, "Item Tag"=w948:string, "dup Tree Parent Tag"=w941:string, "dup Project Tree"=w942:T24)  [unwired: 6 in]
            n492 = call "VIH Project Tree - Sort Items.vi"("error in"=w940, "Recursively (T)"=FALSE, "Parent Tag"=w941, "Project Tree"=w942) -> ("error out"=w939:errorcluster, "dup Project Tree"=w938:T24)  [unwired: 5 in, 1 out]
            n493 = invoke on="Invoke Node" class="Tree (strict)" method="Open/Close.Ensure Visible"(reference=w938, error in=w939, "tag"=w948) -> (reference out=w955:T24, error out=w954:errorcluster)  [unwired: 1 in, 2 out]
            n494 = Build Array(w948) -> (w956:string[])
            n495 = property on="Property Node" class="Tree (strict)"(reference=w955, error in=w954, "Value"=w956) -> (reference out=w957:T24)  [unwired: 1 out]
            n496 = property class="Tree (strict)"(reference=w957, "Active Item Tag"=w948) -> (reference out=w953:T24, "Active Item Row Number"=w951:i32)  [unwired: 1 in, 1 out]
            n497 = Bundle("Active Item Row Number"=w951, 0) -> (w950:cluster{"Active Item Row Number":i32, i32})  [unwired: 1 in]
            n498 = property class="Tree (strict)"(reference=w953, "Key Focus"=TRUE, "EditPos"=w950) -> ()  [unwired: 1 in, 2 out]
          }
          frame "Remove" {
            (unwired) TRUE
            n499 = property on="%Toolbar_Delete" class="Bool"() -> ("DisabledEnum"=w960:T12)  [unwired: 2 in, 2 out]
            n500 = Equal To 0?(x=w960) -> (x = 0?=w959:bool)
            n501 = case shown="True" w959 {
              tunnel: [_ w966] -> w962
              tunnel: w961 -> [_ w965]
              frame False {
                n502 = call <vilib>:"Beep.vi"() -> ()  [unwired: 12 in]
              }
              frame True {
                n503 = Two Button Dialog(message="Remove the selected item(s) from the project.\n\nAre you sure?") -> (T button?=w963:bool)  [unwired: 2 in]
                n504 = case shown="True" w963 {
                  tunnel: [_ "Defer FP Update = ON;\nUpdate Controls;\nUpdate Toolbar: Warning;\nDefer FP Update = OFF;" ("format string")] -> w966
                  tunnel: w965 -> [_ w969]
                  frame False {
                  }
                  frame True {
                    n505 = property class="Tree (strict)"(reference=w969) -> (reference out=w968:refnum<vi>, "Value"=w967:string[])  [unwired: 1 in, 1 out]
                    n506 = call "VIH Project Tree - Delete Items.vi"("Tree Item Tags"=w967, "Project Tree"=w968) -> ("dup Project Tree"=w971:T24)  [unwired: 8 in, 1 out]
                    n507 = property class="Tree (strict)"(reference=w971, "Value"=string[] []) -> ()  [unwired: 1 in, 2 out]
                  }
                }
              }
            }
          }
          frame "Copy File Spec" {
            n508 = property class="Tree (strict)"(reference=w978) -> ("Value"=w977:string[])  [unwired: 1 in, 2 out]
            n509 = for {
              tunnel: w977 -> [w981] mode=indexing
              tunnel: [w980] -> w975 mode=indexing
              n510 = call "VIH Project Tree - Item Tag - Parse.vi"("Tree Item Tag"=w981) -> ("Item File Path"=w980:path)  [unwired: 8 in, 2 out]
            }
            n511 = call "VIH XML - File Array to-from XML String.vi"("cmd (check)"=enum16{"check", "parse", "format"}."format", "Files in"=w975) -> ("available"=w974:bool, "XML out"=w973:string)  [unwired: 6 in, 2 out]
            n512 = case shown="True" w974 {
              tunnel: w973 -> [_ w979]
              frame False {
                n513 = call <vilib>:"Beep.vi"() -> ()  [unwired: 12 in]
              }
              frame True {
                n514 = invoke class="App" method="Clipboard.Write"("Param 0"=w979) -> ()  [unwired: 3 in, 4 out]
              }
            }
          }
          frame "Paste File Spec" {
            n515 = Index Array(array=w987) -> (element=w988:string)  [unwired: 1 in]
            n516 = invoke class="App" method="Clipboard.Read"() -> ("Read Clipbrd"=w985:string)  [unwired: 3 in, 2 out]
            n517 = call "VIH Project Tree - Find Group to Add Item.vi"("Item Tag"=w988, "Project Tree"=w990) -> ("Item Tag (Group)"=w986:string, "dup Project Tree"=w989:T24)  [unwired: 7 in, 1 out]
            n518 = call "VIH XML - File Array to-from XML String.vi"("cmd (check)"=enum16{"check", "parse", "format"}."parse", "XML in"=w985) -> ("available"=w982:bool, "Files out"=w983:path[])  [unwired: 6 in, 2 out]
            n519 = case shown="True" w982 {
              tunnel: w989 -> [_ w999]
              tunnel: [_ "Defer FP Update = ON;\nUpdate Controls;\nDefer FP Update = OFF;" ("format string")] -> w991
              tunnel: w986 -> [_ w993]
              tunnel: w983 -> [_ w992]
              frame False {
                n520 = call <vilib>:"Beep.vi"() -> ()  [unwired: 12 in]
              }
              frame True {
                n521 = call "VIH Project Tree - Add Files.vi"("Ena dialog message (F)"=TRUE, "File Paths"=w992, "Tree Parent Tag"=w993, "Project Tree"=w999) -> ("error out"=w1000:errorcluster, "Top-level Item Tags"=w997:string[], "dup Project Tree"=w995:T24)  [unwired: 4 in, 1 out]
                n522 = Empty Array?(array=w997) -> (empty?=w996:bool)
                n523 = case shown="False" w996 {
                  tunnel: w1000 -> [w1005 _]
                  tunnel: w997 -> [w1003 _]
                  tunnel: w995 -> [w1004 _]
                  frame False {
                    n524 = call "VIH Project Tree - Create Unique Output Names for Added Files.vi"("error in"=w1005, "Added Item Tags"=w1003, "Project Tree"=w1004) -> ("error out"=w1002:errorcluster, "dup Project Tree"=w1001:T24)  [unwired: 7 in]
                    n525 = property class="Tree (strict)"(reference=w1001, error in=w1002, "Value"=w1003) -> (reference out=w1008:T24, error out=w1006:errorcluster)
                    n526 = Index Array(array=w1003) -> (element=w1007:string)  [unwired: 1 in]
                    n527 = invoke class="Tree (strict)" method="Open/Close.Ensure Visible"(reference=w1008, error in=w1006, "tag"=w1007) -> ()  [unwired: 1 in, 4 out]
                  }
                  frame True {
                  }
                }
              }
            }
          }
          frame "----------------------------- 3" {
          }
          frame "CHM Project" {
            n528 = call "VIH Dialog - Compiled HTML Help  Project.vi"("Project Tree"=w1010) -> ()  [unwired: 11 in]
          }
          frame "Open CHM" {
            n529 = call "VIH Project - Container - HHP Generation.vi"() -> ("HHP_Generation out"=w1023:T34)  [unwired: 11 in]
            n530 = Array Size(array=w1022) -> (size(s)=w1021:i32)
            n531 = call "VIH - CHM Project - Get Actual HHP_Generation Params.vi"("HHP_Generation"=w1023) -> ("CHM File Absolute Path"=w1020:path, "HHP_Generation out"=w1018:T34)  [unwired: 8 in, 1 out]
            n532 = Unbundle By Name(w1018) -> ("HHP_Target_CustomPath"=w1016:path)
            n533 = call "VIH HelpGen - FILE - Check File Path (Buffered).vi"("File Path"=w1020) -> ("Good path"=w1012:bool, "dup File Path"=w1019:path)  [unwired: 9 in]
            n534 = call "VIH Utility - FILE - Get and Replace Extension (File Path).vi"("new extension (none)"="txt", "file path"=w1016) -> ("new file path"=w1015:path)  [unwired: 8 in, 1 out]
            n535 = case shown="1" w1021 {
              tunnel: w1022 -> [_ w1037]
              tunnel: [_ w1036] -> w1011
              tunnel: w1015 -> [_ w1035]
              tunnel: w1014 -> [_ w1031]
              frame Default {
              }
              frame 1 {
                # "read Help Info File"
                n536 = Index Array(array=w1037) -> (element=w1038:string)  [unwired: 1 in]
                n537 = To Upper Case(1:w1031) -> (0:w1030:string)
                n538 = Equal?(x=w1030, y="SEL") -> (x = y?=w1028:bool)
                n539 = call "VIH Project Tree - Item Tag - Parse.vi"("Tree Item Tag"=w1038) -> ("Item File Path"=w1034:path)  [unwired: 8 in, 2 out]
                n540 = Empty String/Path?(string/path=w1034) -> (empty?=w1033:bool)
                n541 = Not(x=w1033) -> (.not. x?=w1032:bool)
                n542 = And(x=w1028, y=w1032) -> (x .and. y?=w1027:bool)
                n543 = case shown="True" w1027 {
                  tunnel: w1034 -> [_ w1045]
                  tunnel: [_ w1040] -> w1036
                  tunnel: w1035 -> [_ w1039]
                  frame False {
                  }
                  frame True {
                    n544 = call <vilib>:"Open Config Data.vi"("create file if necessary (T)"=FALSE, "configuration file path"=w1039) -> ("error out"=w1048:errorcluster, "refnum"=w1052:T28)  [unwired: 7 in, 1 out]
                    n545 = call <vilib>:"Get Section Names.vi"("error in (no error)"=w1048, "refnum"=w1052) -> ("error out"=w1049:errorcluster, "section names"=w1047:string[], "refnum out"=w1050:T28)  [unwired: 7 in]
                    n546 = for {
                      shift-right: [w1057] -> w1043
                      shift-left: w1050 -> [w1066]
                      shift-right: [w1056] -> w1042
                      shift-left: w1049 -> [w1065]
                      tunnel: w1047 -> [w1058] mode=indexing
                      tunnel: "Original Path" -> [w1063]
                      tunnel: w1045 -> [w1062]
                      tunnel: "CHM LocalPath" -> [w1055]
                      tunnel: [w1054] -> w1040
                      stop <- w1053 stop-if-true
                      n547 = call-poly <vilib>:"Read Key.vi"("section"=w1058, "error in (no error)"=w1065, "default value"=path "", "key"=w1063, "refnum"=w1066) -> ("error out"=w1059:errorcluster, "value"=w1061:path, "refnum out"=w1060:T28)  [unwired: 3 in, 1 out]
                      n548 = Equal?(x=w1061, y=w1062) -> (x = y?=w1053:bool)
                      n549 = case shown="True" w1053 {
                        tunnel: w1060 -> [w1068 w1077]
                        tunnel: w1059 -> [w1067 w1076]
                        tunnel: w1058 -> [_ w1075]
                        tunnel: [w1068 w1074] -> w1057
                        tunnel: [w1067 w1073] -> w1056
                        tunnel: w1055 -> [_ w1072]
                        tunnel: [_ w1070] -> w1054
                        frame False {
                        }
                        frame True {
                          n550 = call-poly <vilib>:"Read Key.vi"("read raw string? (F)"=TRUE, "section"=w1075, "error in (no error)"=w1076, "default value"="", "key"=w1072, "refnum"=w1077) -> ("error out"=w1073:errorcluster, "value"=w1070:string, "refnum out"=w1074:T28)  [unwired: 2 in, 1 out]
                        }
                      }
                    }
                    n551 = call <vilib>:"Close Config Data.vi"("error in (no error)"=w1042, "write file if changed (T)"=FALSE, "refnum"=w1043) -> ()  [unwired: 7 in, 2 out]
                  }
                }
              }
            }
            n552 = case shown="True" w1012 {
              tunnel: w1019 -> [_ w1026]
              tunnel: w1011 -> [_ w1025]
              frame False {
                n553 = call <vilib>:"Beep.vi"() -> ()  [unwired: 12 in]
              }
              frame True {
                n554 = call "VIH Utility - HELP - Open Help File.vi"("Topic"=w1025, "Help Path"=w1026) -> ("error out"=w1024:errorcluster)  [unwired: 8 in, 1 out]
                n555 = call <vilib>:"Simple Error Handler.vi"("error in (no error)"=w1024) -> ()  [unwired: 4 in, 5 out]
              }
            }
          }
          frame "----------------------------- 4" {
          }
          frame "Settings" {
            n556 = call "VIH Dialog - Settings.vi"() -> ()  [unwired: 11 in, 1 out]
          }
          frame "----------------------------- 5" {
          }
          frame "Help" {
            n557 = call "VIH Constant - Help Folder.vi"("append path"=path "VIHelpeks.chm" ("Path")) -> ("Help path"=w1079:path)  [unwired: 10 in]
            n558 = call "VIH Utility - HELP - Open Help File.vi"("Help Path"=w1079) -> ("error out"=w1078:errorcluster)  [unwired: 9 in, 1 out]
            n559 = call <vilib>:"Simple Error Handler.vi"("error in (no error)"=w1078) -> ()  [unwired: 4 in, 5 out]
          }
          frame "About" {
            n560 = call "VIH Dialog - About.vi"() -> ()  [unwired: 11 in, 1 out]
          }
        }
        n561 = Concatenate Strings(w622, w630) -> (w623:string)
      }
      frame "EXEC" {
        n562 = Format Into String(format string="Set Busy = ON;\nKey Focus = Tree;\n\n%s;\n\nSet Busy = OFF;\nKey Focus = Tree;", w1084) -> (resulting string=w1083:string)  [unwired: 2 in, 1 out]
        n563 = Concatenate Strings(w1083, w1081) -> (w1082:string)
      }
      frame "------------------------------- 2" {
      }
      frame "Ask to Save Project" {
        n564 = call "VIH Project - Change Flag.vi"() -> ("Flag"=w1090:bool)  [unwired: 10 in, 1 out]
        n565 = call "VIH Project - Container - Project File Path.vi"() -> ("It's example"=w1087:bool)  [unwired: 9 in, 2 out]
        n566 = Not(x=w1087) -> (.not. x?=w1088:bool)
        n567 = And(x=w1090, y=w1088) -> (x .and. y?=w1089:bool)
        n568 = case shown="True" w1089 {
          tunnel: w1092 -> [w1093 w1096]
          tunnel: [w1093 w1095] -> w1091
          frame False {
          }
          frame True {
            n569 = call <vilib>:"Three Button Dialog.vi"("Keyboard Shortcuts (Left is <Enter>)"=T9 {"Left Button Key Shortcut"={"Control"=FALSE, "Shift"=FALSE, "Key"="<Enter>"}, "Center Button Key Shortcut"={"Control"=FALSE, "Shift"=FALSE, "Key"=""}, "Right Button Key Shortcut"={"Control"=FALSE, "Shift"=FALSE, "Key"="<Escape>"}}, "Window Title (\"\")"="Save Project?" ("Window Title (\"\")"), "Right Button Text (\"Cancel\")"="Cancel           " ("Right Button Text (\"Cancel\")"), "Center Button Text (\"No\")"="Don't Save     " ("Center Button Text (\"No\")"), "Left Button Text (\"Yes\")"="Save              " ("Left Button Text (\"Yes\")"), "message"="The project has unsaved changes. Would you like to save changes?") -> ("Which Button?"=w1097:T35)  [unwired: 5 in]
            n570 = case shown="\"Left Button\"" w1097 {
              tunnel: w1096 -> [w1106 w1107 _ _]
              tunnel: [w1105 w1107 _ _] -> w1095
              tunnel: "Project = Save;" -> [w1104 _ _ _]
              frame "Left Button" {
                n571 = Concatenate Strings(w1104, w1106) -> (w1105:string)
              }
              frame "Center Button" {
              }
              frame "Right Button" {
              }
              frame "Window Close" {
              }
            }
          }
        }
      }
      frame "Ask to Save Lost Rules" {
        n572 = control-ref of="Tree"() -> (w1112:refnum<vi>)
        n573 = call "VIH Project Tree - Find Lost Item Rules.vi"("Project Tree"=w1112) -> ("Lost Rules (Owner Paths)"=w1110:path[])  [unwired: 8 in, 2 out]
        n574 = Empty Array?(array=w1110) -> (empty?=w1111:bool)
        n575 = case shown="False" w1111 {
          selector: w1111 -> [_ w1134]
          tunnel: [w1119 w1134] -> w1113
          tunnel: w1110 -> [w1118 _]
          tunnel: [w1117 _] -> w1108
          frame False {
            n576 = call <vilib>:"Three Button Dialog.vi"("Keyboard Shortcuts (Left is <Enter>)"=T9 {"Left Button Key Shortcut"={"Control"=FALSE, "Shift"=FALSE, "Key"="<Enter>"}, "Center Button Key Shortcut"={"Control"=FALSE, "Shift"=FALSE, "Key"=""}, "Right Button Key Shortcut"={"Control"=FALSE, "Shift"=FALSE, "Key"="<Escape>"}}, "Window Title (\"\")"="Save Lost Rules?" ("Window Title (\"\")"), "Right Button Text (\"Cancel\")"="Cancel       " ("Right Button Text (\"Cancel\")"), "Center Button Text (\"No\")"="No             " ("Center Button Text (\"No\")"), "Left Button Text (\"Yes\")"="Yes            " ("Left Button Text (\"Yes\")"), "message"="There are lost file rules in the project. Would you like to save the lost rules in the project file?") -> ("Which Button?"=w1120:T35)  [unwired: 5 in]
            n577 = case shown="\"Center Button\"" w1120 {
              tunnel: [TRUE TRUE FALSE] -> w1119
              tunnel: w1118 -> [_ w1129 _]
              tunnel: [_ "Update Toolbar: Warning;" _] -> w1117
              frame "Left Button" {
              }
              frame "Center Button" {
                n578 = for {
                  tunnel: w1129 -> [w1131] mode=indexing
                  n579 = call "VIH Project - Container - Item Rules.vi"("cmd (get)"=T10."delete", "Item Path"=w1131) -> ()  [unwired: 5 in, 5 out]
                }
              }
              frame "Right Button", "Window Close" {
              }
            }
          }
          frame True {
          }
        }
        n580 = Select(t=w1116, s=w1113, f="Update Toolbar: Warning;\nDefer FP Update = OFF;\nSet Busy = OFF;\nKey Focus = Tree;") -> (s? t:f=w1115:string)
        n581 = Concatenate Strings(w1108, w1115) -> (w1109:string)
      }
      frame "------------------------------- 3" {
      }
      frame "Project" {
        n582 = Match Pattern(string=w1145, regular expression="\\?") -> (before substring=w1143:string, after substring=w1142:string)  [unwired: 1 in, 2 out]
        n583 = call <vilib>:"Trim Whitespace.vi"("string"=w1143) -> ("trimmed string"=w1141:string)  [unwired: 1 in]
        n584 = call <vilib>:"Trim Whitespace.vi"("string"=w1142) -> ("trimmed string"=w1139:string)  [unwired: 1 in]
        n585 = case shown="\"Save\"" w1141 {
          tunnel: w1140 -> [w1147 _ _ _]
          tunnel: w1139 -> [_ _ w1152 w1188]
          tunnel: "*.hgprj" ("pattern (all files)") -> [_ _ w1156 w1182]
          tunnel: [w1146 w1149 w1153 w1173] -> w1137
          tunnel: w1136 -> [w1146 w1150 w1155 w1177]
          frame Default {
            n586 = One Button Dialog(message=w1147) -> ()  [unwired: 1 in, 1 out]
          }
          frame "New" {
            n587 = Concatenate Strings("Ask to Save Project;\n\nProject: New;" ("t"), w1150) -> (w1149:string)
          }
          frame "Open" {
            n588 = case shown="\"OK\"" w1152 {
              tunnel: w1156 -> [_ w1159]
              tunnel: [w1157 w1158] -> w1154
              tunnel: "Ask to Save Project;\n\nProject = Open ? OK;" -> [w1157 _]
              frame Default {
              }
              frame "OK" {
                n589 = call "File Dialog"("prompt"="Open Project", "pattern (all files)"=w1159) -> ("selected path"=w1162:path, "error out"=w1163:errorcluster)  [unwired: 10 in, 2 out]
                n590 = Format Into String(format string="Set Busy = ON;\n\nProject: Load XML = %s;\n\nSet Busy = OFF;", initial string="", error in=w1163, w1162) -> (resulting string=w1158:string)  [unwired: 1 out]
              }
            }
            n591 = Concatenate Strings(w1154, w1155) -> (w1153:string)
          }
          frame "Save" {
            (unwired) ""
            n592 = call "VIH Project - Container - Project File Path.vi"() -> ("Project File Path"=w1171:path, "It's example"=w1168:bool)  [unwired: 9 in, 1 out]
            n593 = To Upper Case(1:w1188) -> (0:w1187:string)
            n594 = And(x=w1168, y=TRUE) -> (x .and. y?=w1166:bool)
            n595 = Search/Split String(string=w1182, search string/char (-)=".") -> (match + rest of string=w1180:string)  [unwired: 1 in, 2 out]
            n596 = call "VIH Utility - FILE - Get Path Attributes (Empty-NAP-Rel).vi"("Path"=w1171) -> ("Not A Path or Empty path"=w1169:bool, "dup Path"=w1170:path)  [unwired: 6 in, 3 out]
            n597 = Equal?(x=w1187, y="AS") -> (x = y?=w1185:bool)
            n598 = Or(x=w1169, y=w1166) -> (x .or. y?=w1167:bool)
            n599 = Concatenate Strings("My Project", w1180) -> (w1178:string)
            n600 = Or(x=w1185, y=w1167) -> (x .or. y?=w1184:bool)
            n601 = case shown="True" w1184 {
              tunnel: [_ w1199] -> w1175
              tunnel: [w1191 w1198] -> w1190
              tunnel: w1170 -> [w1191 w1194]
              tunnel: w1167 -> [_ w1195]
              tunnel: w1182 -> [_ w1193]
              tunnel: w1178 -> [_ w1192]
              frame False {
              }
              frame True {
                n602 = case shown="False" w1195 {
                  tunnel: [w1203 _] -> w1197
                  tunnel: [w1202 w1204] -> w1196
                  tunnel: w1194 -> [w1201 _]
                  tunnel: w1192 -> [_ w1204]
                  frame False {
                    n603 = Strip Path(path=w1201) -> (stripped path=w1203:path, name=w1202:string)
                  }
                  frame True {
                  }
                }
                n604 = call "VIH Utility - FILE - Save File Dialog.vi"("pattern"=w1193, "prompt"="Save Project", "default name"=w1196, "start path"=w1197) -> ("error out"=w1199:errorcluster, "File path"=w1198:path)  [unwired: 5 in, 1 out]
              }
            }
            n605 = Format Into String(format string="Set Busy = ON;\n\nAsk to Save Lost Rules;\nProject: Save XML = %s;\n\nSet Busy = OFF;", initial string="", error in=w1175, w1190) -> (resulting string=w1176:string)  [unwired: 1 out]
            n606 = Concatenate Strings(w1176, w1177) -> (w1174:string)
            n607 = Select(t="Defer FP Update = OFF;\nSet Busy = OFF;\nKey Focus = Tree;", s=w1175, f=w1174) -> (s? t:f=w1173:string)
          }
        }
      }
      frame "Example", "RecentProjects" {
        n608 = Format Into String(format string="Ask to Save Project;\n\nSet Busy = ON;\n\nProject: Load XML = %s;\n\nSet Busy = OFF;", initial string="", w1205) -> (resulting string=w1208:string)  [unwired: 1 in, 1 out]
        n609 = Concatenate Strings(w1208, w1210) -> (w1209:string)
      }
      frame "Project: New" {
        n610 = case shown="Default" w1212 {
          tunnel: [enum32{"Default", "JSBased"}."Default" ("Project Type out") w1238] -> w1213
          tunnel: [TRUE w1237] -> w1211
          frame "Silent" {
          }
          frame Default {
            n611 = call "VIH Dialog - ProjectType.vi"() -> ("OK out"=w1237:bool, "Project Type out"=w1238:enum32{"Default", "JSBased"})  [unwired: 10 in]
          }
        }
        n612 = case shown="True" w1211 {
          tunnel: [_ "Set Busy = ON;\nDefer FP Update = ON;\n\nTree: New;\n\nUpdate Window Title;\nUpdate Controls = INIT;\nUpdate Toolbar: Warning;\n\nDefer FP Update = OFF;\nSet Busy = OFF;\n\nKey Focus = Tree;"] -> w1214
          tunnel: w1213 -> [_ w1218]
          frame False {
          }
          frame True {
            n613 = flat-sequence {
              tunnel: w1218 -> [w1222]
              tunnel: [w1224] -> w1217
              tunnel: w1217 -> [w1231]
              frame #0 {
                n614 = case shown="\"JSBased\"" w1222 {
                  tunnel: [w1227 w1228] -> w1224
                  frame "Default" {
                    n615 = call "VIH Project - New Project - Master Rule (Default).vi"() -> ("Master Rule"=w1227:T15)  [unwired: 10 in, 1 out]
                  }
                  frame "JSBased" {
                    n616 = call "VIH Project - New Project - Master Rule (JS Based).vi"() -> ("Master Rule"=w1228:T15)  [unwired: 10 in, 1 out]
                  }
                }
                n617 = call "VIH HelpGen - FILE - Check File Path (Buffered).vi"("cmd (get)"=enum16{"Init", "get"}."Init") -> ()  [unwired: 9 in, 2 out]
                n618 = call "VIH Project - Container - HHP Generation.vi"("cmd (get)"=enum16{"get", "set"}."set") -> ()  [unwired: 10 in, 1 out]
                n619 = call "VIH Project - Container - Product Info.vi"("cmd (get)"=enum16{"get", "set"}."set") -> ()  [unwired: 10 in, 1 out]
                n620 = call "VIH Project - Container - Project File Path.vi"("cmd (get)"=enum16{"get", "set"}."set", "Project File Path in"=path "") -> ()  [unwired: 7 in, 3 out]
              }
              frame #1 {
                n621 = call "VIH Project - Container - Item Rules.vi"("cmd (get)"=T10."Init") -> ()  [unwired: 6 in, 5 out]
                n622 = call "VIH Project - Container - Group Rules.vi"("cmd (get)"=T11."Init") -> ()  [unwired: 6 in, 5 out]
                n623 = call "VIH Project - Container - Master Rule.vi"("cmd (get)"=enum16{"get", "set"}."set", "Rule in"=w1231) -> ()  [unwired: 9 in, 1 out]
              }
              frame #2 {
                n624 = call "VIH Constant - Temporal Build Log File.vi"() -> ("Temporal Build Log File"=w1233:path)  [unwired: 11 in]
                n625 = Delete(path (use dialog)=w1233) -> ()  [unwired: 4 in, 3 out]
                n626 = call "VIH Project - Change Flag.vi"("cmd (get)"=enum16{"get", "set", "reset"}."reset") -> ()  [unwired: 9 in, 2 out]
              }
            }
          }
        }
        n627 = Concatenate Strings(w1214, w1216) -> (w1215:string)
      }
      frame "Project: Load XML" {
        n628 = String To Path(string=w1283) -> (path=w1268:path)
        n629 = call "VIH Project - Container - Project File Path.vi"("cmd (get)"=enum16{"get", "set"}."set", "Project File Path in"=w1268) -> ("Project File Path"=w1250:path, "It's example"=w1239:bool)  [unwired: 7 in, 1 out]
        n630 = Format Into String(format string=" - Loadiing \"%s\"", initial string=w1253, w1250) -> (resulting string=w1251:string)  [unwired: 1 in, 1 out]
        n631 = Strip Path(path=w1250) -> (stripped path=w1262:path)  [unwired: 1 out]
        n632 = property class="VI"("Front Panel.Title"=w1251) -> (error out=w1249:errorcluster)  [unwired: 2 in, 1 out]
        n633 = call <vilib>:"Clear Errors.vi"("error in (no error)"=w1249) -> ("error out"=w1248:errorcluster)  [unwired: 5 in, 1 out]
        n634 = call "VIH ProjFile - Core.vi"("cmd (get)"=enum16{"get", "create", "load", "save", "close"}."load", "error in"=w1248, "Project file"=w1250) -> ("error out"=w1281:errorcluster, "Project"=w1280:T36)  [unwired: 7 in]
        n635 = Unbundle By Name(w1280) -> ("Project"=w1270:refnum<k20>)
        n636 = Unbundle By Name(w1280) -> ("DOM doc"=w1282:refnum<k20>)
        n637 = call "VIH ProjFile - Group Rule - Read.vi"("MasterRule (F)"=TRUE, "error in"=w1281, "Project Folder"=w1262, "XML Parent Item"=w1270) -> ("error out"=w1279:errorcluster, "Group Rule out"=w1241:T15, "changed"=w1240:bool, "dup XML Parent Item"=w1278:refnum<k20>)  [unwired: 4 in]
        n638 = invoke class="Document" method="DUXGetXMLPP"(reference=w1282) -> ("XML"=w1273:string)  [unwired: 3 in, 3 out]
        n639 = call "VIH Project - Container - Group Rules.vi"("cmd (get)"=T11."Init") -> ("error out"=w1271:errorcluster)  [unwired: 6 in, 4 out]
        n640 = call "VIH ProjFile - Item Rule Array - Read.vi"("Project Folder"=w1262, "error in"=w1279, "XML Parent Item"=w1278) -> ("error out"=w1264:errorcluster, "Item Rules"=w1274:T30[], "Item Paths"=w1275:path[], "dup XML Parent Item"=w1265:refnum<k20>)  [unwired: 5 in]
        n641 = Unbundle By Name(w1241) -> ("Build Root Dir"=w1259:path)
        n642 = call "VIH Project - Container - Item Rules.vi"("cmd (get)"=T10."Init", "error in"=w1271) -> ("error out"=w1277:errorcluster)  [unwired: 5 in, 4 out]
        n643 = call "VIH HelpGen - FILE - Check File Path (Buffered).vi"("cmd (get)"=enum16{"Init", "get"}."Init") -> ()  [unwired: 9 in, 2 out]
        n644 = call "VIH UI - Project XML Indicator.vi"("XML in"=w1273) -> ()  [unwired: 11 in]
        n645 = for {
          tunnel: w1277 -> [w1293]
          tunnel: w1275 -> [w1292] mode=indexing
          tunnel: w1274 -> [w1291] mode=indexing
          n646 = call "VIH Project - Container - Item Rules.vi"("cmd (get)"=T10."set", "error in"=w1293, "Item Rule"=w1291, "Item Path"=w1292) -> ()  [unwired: 3 in, 5 out]
        }
        n647 = call "VIH Project - Container - Master Rule.vi"("cmd (get)"=enum16{"get", "set"}."set", "Rule in"=w1241) -> ()  [unwired: 9 in, 1 out]
        n648 = call "VIH ProjFile - HHP Generation - Read.vi"("error in"=w1264, "Build Root Folder"=w1259, "Project Folder"=w1262, "XML Parent Item"=w1265) -> ("error out"=w1257:errorcluster, "HHP_Generation out"=w1261:T34, "dup XML Parent Item"=w1256:refnum<k20>)  [unwired: 5 in]
        n649 = call "VIH ProjFile - Product Info - Read.vi"("error in"=w1257, "XML Parent Item"=w1256) -> ("error out"=w1255:errorcluster, "Product Info out"=w1254:T37)  [unwired: 7 in, 1 out]
        n650 = call "VIH Project - Container - HHP Generation.vi"("cmd (get)"=enum16{"get", "set"}."set", "HHP_Generation in"=w1261) -> ()  [unwired: 9 in, 1 out]
        n651 = call "VIH Project - Container - Product Info.vi"("cmd (get)"=enum16{"get", "set"}."set", "Product Info in"=w1254) -> ()  [unwired: 9 in, 1 out]
        n652 = call <vilib>:"Simple Error Handler.vi"("error in (no error)"=w1255) -> ("error out"=w1263:errorcluster)  [unwired: 4 in, 4 out]
        n653 = Select(t="changed", s=w1240, f="") -> (s? t:f=w1245:string)
        n654 = case shown="False" w1239 {
          tunnel: w1250 -> [w1287 _]
          tunnel: w1263 -> [_ _]
          frame False {
            n655 = Current VI's Menubar() -> (w1288:refnum<k9>)
            n656 = call "VIH Utility - MENU - Recent Paths Handler.vi"("cmd (get list)"=enum32{"get list", "delete", "insert"}."insert", "Path"=w1287, "menubar"=w1288) -> ()  [unwired: 5 in, 4 out]
          }
          frame True {
          }
        }
        n657 = Format Into String(format string="Defer FP Update = ON;\n\nTree: New;\nTree: Build;\n\nProject: Close XML = %s;\n\nUpdate Window Title;\nUpdate Controls = INIT;\nUpdate Toolbar: Warning = Dialog;\n\nDefer FP Update = OFF;\n\nKey Focus = Tree;\n\nTree: Check;", w1245) -> (resulting string=w1246:string)  [unwired: 2 in, 1 out]
        n658 = Concatenate Strings(w1246, w1286) -> (w1285:string)
      }
      frame "Project: Save XML" {
        (unwired) "Project: Close XML;\n\nUpdate Window Title;\nUpdate Toolbar;\nUpdate Toolbar: Warning;"  # Project: Close XML;  Update Window Title; Update Toolbar; Update Toolbar: Warning;
        n659 = String To Path(string=w1327) -> (path=w1307:path)
        n660 = call "VIH ProjFile - Core.vi"("cmd (get)"=enum16{"get", "create", "load", "save", "close"}."create") -> ("error out"=w1296:errorcluster, "Project"=w1310:T36)  [unwired: 9 in]
        n661 = control-ref of="Tree"() -> (w1324:refnum<vi>)
        n662 = call "VIH Project - Container - Project File Path.vi"("cmd (get)"=enum16{"get", "set"}."set", "Project File Path in"=w1307) -> ("Project File Path"=w1306:path)  [unwired: 7 in, 2 out]
        n663 = Unbundle By Name(w1310) -> ("DOM doc"=w1322:refnum<k20>, "Project"=w1294:refnum<k20>, "Files"=w1309:refnum<k20>)
        n664 = call "VIH Project - Container - Product Info.vi"() -> ("Product Info out"=w1298:T37)  [unwired: 11 in]
        n665 = call "VIH Project - Container - Item Rules.vi"("cmd (get)"=T10."get all") -> ("error out"=w1315:errorcluster, "Item Paths"=w1314:path[])  [unwired: 6 in, 3 out]
        n666 = call "VIH Project Tree - Item Tag - Build.vi"("Item Type"=VIH_Project_Tree_Typedef_-_Tree_Item_Type."Proj Files") -> ("Tree Item Tag"=w1317:string)  [unwired: 9 in, 1 out]
        n667 = Array Size(array=w1314) -> (size(s)=w1316:i32)
        n668 = call "VIH ProjFile - Product Info - Write.vi"("error in"=w1296, "Product Info"=w1298, "XML Parent Item"=w1294) -> ("error out"=w1295:errorcluster)  [unwired: 7 in, 1 out]
        n669 = for {
          N: w1316 -> [_]
          tunnel: w1315 -> [w1333]
          tunnel: [w1331] -> w1313 mode=indexing
          i -> [w1332]
          n670 = call "VIH Project - Container - Item Rules.vi"("error in"=w1333, "Item Idx (-1)"=w1332) -> ("Item Rule out"=w1331:T30)  [unwired: 5 in, 4 out]
        }
        n671 = Strip Path(path=w1306) -> (stripped path=w1301:path)  [unwired: 1 out]
        n672 = call "VIH Project - Container - Master Rule.vi"() -> ("Rule out"=w1300:T15)  [unwired: 11 in]
        n673 = call "VIH ProjFile - File Tree - Write.vi"("Tree Parent Tag"=w1317, "Project Tree"=w1324, "error in"=w1295, "Project Folder"=w1301, "XML Parent Item"=w1309) -> ("error out"=w1320:errorcluster)  [unwired: 5 in, 1 out]
        n674 = Unbundle By Name(w1300) -> ("Build Root Dir"=w1299:path)
        n675 = call "VIH ProjFile - Group Rule - Write.vi"("MasterRule (F)"=TRUE, "error in"=w1320, "Group Rule"=w1300, "Project Folder"=w1301, "XML Parent Item"=w1294) -> ("error out"=w1318:errorcluster, "dup XML Parent Item"=w1319:refnum<k20>)  [unwired: 5 in]
        n676 = call "VIH ProjFile - Item Rule Array - Write.vi"("Project Folder"=w1301, "error in"=w1318, "Item Rules"=w1313, "Item Paths"=w1314, "XML Parent Item"=w1319) -> ("error out"=w1304:errorcluster, "dup XML Parent Item"=w1303:refnum<k20>)  [unwired: 5 in]
        n677 = call "VIH Project - Container - HHP Generation.vi"() -> ("HHP_Generation out"=w1302:T34)  [unwired: 11 in]
        n678 = call "VIH ProjFile - HHP Generation - Write.vi"("Build Root Dir"=w1299, "Project Folder"=w1301, "error in"=w1304, "HHP_Generation"=w1302, "XML Parent Item"=w1303) -> ("error out"=w1297:errorcluster)  [unwired: 5 in, 1 out]
        n679 = invoke class="Document" method="DUXGetXMLPP"(reference=w1322, error in=w1297) -> ("XML"=w1311:string)  [unwired: 2 in, 3 out]
        n680 = call "VIH ProjFile - Core.vi"("cmd (get)"=enum16{"get", "create", "load", "save", "close"}."save", "error in"=w1297, "Project file"=w1306) -> ("error out"=w1326:errorcluster)  [unwired: 7 in, 1 out]
        n681 = case shown="No Error" w1326 {
          tunnel: w1306 -> [w1334 _]
          frame No Error {
            n682 = Current VI's Menubar() -> (w1335:refnum<k9>)
            n683 = call "VIH Utility - MENU - Recent Paths Handler.vi"("cmd (get list)"=enum32{"get list", "delete", "insert"}."insert", "Path"=w1334, "menubar"=w1335) -> ()  [unwired: 5 in, 4 out]
          }
          frame Error {
          }
        }
        n684 = call "VIH UI - Project XML Indicator.vi"("XML in"=w1311) -> ()  [unwired: 11 in]
        n685 = Concatenate Strings("Project: Close XML;\n\nUpdate Window Title;\nUpdate Controls;\nUpdate Toolbar: Warning;", w1330) -> (w1329:string)
      }
      frame "Project: Close XML" {
        n686 = call "VIH ProjFile - Core.vi"("cmd (get)"=enum16{"get", "create", "load", "save", "close"}."close") -> ()  [unwired: 9 in, 2 out]
        n687 = call "VIH Project - Change Flag.vi"("cmd (get)"=enum16{"get", "set", "reset"}."reset") -> ("Flag"=w1338:bool)  [unwired: 9 in, 1 out]
        n688 = case shown="\"changed\"" w1337 {
          tunnel: w1338 -> [_ _]
          frame Default {
          }
          frame "changed" {
            n689 = call "VIH Project - Change Flag.vi"("cmd (get)"=enum16{"get", "set", "reset"}."set") -> ()  [unwired: 9 in, 2 out]
          }
        }
      }
      frame "Project: Build" {
        w1363 = path[] []
        # "if empty, build for all"
        n690 = call "VIH Project - Container - Project File Path.vi"() -> ("Project File Path"=w1348:path)  [unwired: 9 in, 2 out]
        n691 = case shown="\"SEL\"" w1367 {
          tunnel: w1368 -> [_ w1462 w1470]
          tunnel: [_ w1460 w1470] -> w1366
          tunnel: [TRUE _ _] -> w1360
          frame "ALL", Default {
          }
          frame "SEL" {
            n692 = control-ref of="Tree"() -> (w1463:refnum<vi>)
            n693 = for {
              tunnel: w1463 -> [w1469]
              tunnel: w1462 -> [w1468] mode=indexing
              shift-right: [w1465] -> w1460
              shift-left: string[] [] -> [w1464]
              n694 = call "VIH Project Tree - Get Tree Item Tags.vi"("Parent Item Tag"=w1468, "Project Tree"=w1469) -> ("Child Item Tags"=w1466:string[], "dup Parent Item Tag"=w1467:string)  [unwired: 6 in, 2 out]
              n695 = Build Array (concatenate)(w1464, w1467, w1466) -> (w1465:string[])
            }
          }
          frame "SELONLY" {
          }
        }
        n696 = Strip Path(path=w1348) -> (name=w1349:string)  [unwired: 1 out]
        n697 = Format Into String(format string=" - Building \"%s\"", initial string=w1344, w1349) -> (resulting string=w1346:string)  [unwired: 1 in, 1 out]
        n698 = property class="VI"("Front Panel.Title"=w1346) -> (error out=w1345:errorcluster)  [unwired: 2 in, 1 out]
        n699 = call <vilib>:"Clear Errors.vi"("error in (no error)"=w1345) -> ("error out"=w1343:errorcluster)  [unwired: 5 in, 1 out]
        n700 = property on="Tree" class="Tree (strict)"(error in=w1343) -> ("All Tags"=w1364:string[])  [unwired: 1 in, 2 out]
        n701 = for {
          tunnel: w1364 -> [w1379] mode=indexing
          shift-right: [w1383] -> w1358
          shift-left: w1363 -> [w1384]
          shift-right: [w1381] -> w1357
          shift-left: w1363 -> [w1382]
          tunnel: w1366 -> [w1378]
          shift-right: [w1375] -> w1361
          shift-left: w1363 -> [w1377]
          n702 = call "VIH Project Tree - Item Tag - Parse.vi"("Tree Item Tag"=w1379) -> ("Item File Path"=w1385:path, "Item Type"=w1386:T2)  [unwired: 8 in, 1 out]
          n703 = case shown="\"Project\"" w1386 {
            tunnel: w1385 -> [w1398 _ _ _ _ _ w1422 _ w1428 w1432 w1435 w1439 w1442 w1445 w1449 w1452 w1456]
            tunnel: w1384 -> [w1402 w1413 w1415 w1417 w1419 w1421 w1425 w1427 w1431 w1434 w1438 w1441 w1444 w1448 w1451 w1455 w1458]
            tunnel: [w1401 w1413 w1415 w1417 w1419 w1421 w1425 w1427 w1430 w1434 w1438 w1441 w1444 w1448 w1451 w1455 w1458] -> w1383
            tunnel: w1382 -> [w1399 w1412 w1414 w1416 w1418 w1420 w1424 w1426 w1429 w1433 w1437 w1440 w1443 w1447 w1450 w1454 w1457]
            tunnel: [w1400 w1412 w1414 w1416 w1418 w1420 w1423 w1426 w1429 w1433 w1436 w1440 w1443 w1446 w1450 w1453 w1457] -> w1381
            tunnel: [w1398 _ _ _ _ _ w1422 _ w1428 w1432 w1435 w1439 w1442 w1445 w1449 w1452 w1456] -> w1376
            frame "<Invalid>" {
              n704 = call <vilib>:"Get File Extension.vi"("file"=w1398) -> ("lowercase file extension"=w1403:string)  [unwired: 7 in, 3 out]
              n705 = case shown="\"mnu\"" w1403 {
                tunnel: w1402 -> [w1407 w1411]
                tunnel: w1398 -> [_ w1410]
                tunnel: [w1407 w1409] -> w1401
                tunnel: [w1405 w1408] -> w1400
                tunnel: w1399 -> [w1406 w1408]
                tunnel: w1398 -> [w1404 _]
                frame Default {
                  n706 = Build Array (concatenate)(w1406, w1404) -> (w1405:path[])
                }
                frame "mnu" {
                  n707 = Build Array (concatenate)(w1411, w1410) -> (w1409:path[])
                }
              }
            }
            frame "Project" {
            }
            frame "Proj Files" {
            }
            frame "Proj Rules" {
            }
            frame "File Group" {
            }
            frame "Rule Group" {
            }
            frame "Any File" {
              n708 = Build Array (concatenate)(w1424, w1422) -> (w1423:path[])
            }
            frame "LV Func" {
            }
            frame ".mnu" {
              n709 = Build Array (concatenate)(w1431, w1428) -> (w1430:path[])
            }
            frame ".mnu (dyn)" {
            }
            frame ".vi", ".vit", ".ctl", ".ctt" {
              n710 = Build Array (concatenate)(w1437, w1435) -> (w1436:path[])
            }
            frame ".vi (dyn)", ".vit (dyn)" {
            }
            frame ".ctl (dyn)", ".ctt (dyn)" {
            }
            frame "polyVI", "expVI" {
              n711 = Build Array (concatenate)(w1447, w1445) -> (w1446:path[])
            }
            frame "polyVI (dyn)", "expVI (dyn)" {
            }
            frame "HTML" {
              n712 = Build Array (concatenate)(w1454, w1452) -> (w1453:path[])
            }
            frame "PolyVI Inst" {
            }
          }
          n713 = Empty String/Path?(string/path=w1376) -> (empty?=w1380:bool)
          n714 = case shown="False" w1380 {
            tunnel: w1379 -> [w1392 _]
            tunnel: w1378 -> [w1391 _]
            tunnel: w1377 -> [w1390 w1397]
            tunnel: w1376 -> [w1389 _]
            tunnel: [w1388 w1397] -> w1375
            frame False {
              n715 = Search 1D Array(1D array=w1391, element=w1392) -> (index of element=w1387:i32)  [unwired: 1 in]
              n716 = case shown="..-1" w1387 {
                tunnel: w1390 -> [w1393 w1396]
                tunnel: w1389 -> [_ w1395]
                tunnel: [w1393 w1394] -> w1388
                frame ..-1 {
                }
                frame 0.. {
                  n717 = Build Array (concatenate)(w1396, w1395) -> (w1394:path[])
                }
              }
            }
            frame True {
            }
          }
        }
        n718 = control-ref of="Tree"() -> (w1365:refnum<vi>)
        n719 = Concatenate Strings("Update Window Title;\nUpdate Toolbar;" ("string"), w1369) -> (w1351:string)
        n720 = Empty Array?(array=w1361) -> (empty?=w1362:bool)
        n721 = Empty Array?(array=w1357) -> (empty?=w1356:bool)
        n722 = Empty Array?(array=w1358) -> (empty?=w1355:bool)
        n723 = Not(x=w1362) -> (.not. x?=w1359:bool)
        n724 = Not And(1:w1355, 2:w1356) -> (0:w1354:bool)
        n725 = Or(x=w1359, y=w1360) -> (x .or. y?=w1353:bool)
        n726 = And(x=w1354, y=w1353) -> (x .and. y?=w1352:bool)
        n727 = case shown="True" w1352 {
          tunnel: w1365 -> [_ w1374]
          tunnel: w1358 -> [_ w1373]
          tunnel: w1357 -> [_ w1372]
          tunnel: w1361 -> [_ w1371]
          frame False {
            n728 = call <vilib>:"Beep.vi"() -> ()  [unwired: 12 in]
          }
          frame True {
            n729 = call "VIH Dialog - Allow_Optional_Terminals in Context Help.vi"() -> ("error out"=w1370:errorcluster)  [unwired: 11 in]
            n730 = call "VIH HelpGen - Build HTML Help.vi"("Allowed files (empty=all)"=w1371, "error in"=w1370, "File paths"=w1372, "Menu paths"=w1373, "Project Tree"=w1374) -> ()  [unwired: 5 in, 2 out]
          }
        }
      }
      frame "Project: Change Type" {
        n731 = call "VIH Dialog - ProjectType.vi"("Title"="Reconfigure Master Rule") -> ("OK out"=w1475:bool, "Project Type out"=w1474:enum32{"Default", "JSBased"})  [unwired: 9 in]
        n732 = case shown="True" w1475 {
          tunnel: w1474 -> [_ w1488]
          tunnel: ["Key Focus = Tree;" "Set Busy = ON;\nDefer FP Update = ON;\n\nUpdate Window Title;\nUpdate Controls;\nUpdate Toolbar: Warning;\n\nDefer FP Update = OFF;\nSet Busy = OFF;\n\nKey Focus = Tree;"] -> w1472
          frame False {
          }
          frame True {
            n733 = case shown="\"JSBased\"" w1488 {
              tunnel: [w1489 w1490] -> w1486
              frame "Default" {
                n734 = call "VIH Project - New Project - Master Rule (Default).vi"() -> ("Master Rule"=w1489:T15)  [unwired: 10 in, 1 out]
              }
              frame "JSBased" {
                n735 = call "VIH Project - New Project - Master Rule (JS Based).vi"() -> ("Master Rule"=w1490:T15)  [unwired: 10 in, 1 out]
              }
            }
            n736 = Unbundle By Name(w1486) -> ("Source Paths.CSS Files"=w1485:path[], "Source Paths.JS Files"=w1484:path[], "Source Paths.VI Template"=w1483:path, "Source Paths.Menu Template"=w1482:path, "Source Paths.PolyVI Template"=w1481:path)
            n737 = call "VIH Project - Container - Master Rule.vi"() -> ("Rule out"=w1487:T15)  [unwired: 11 in]
            n738 = Bundle By Name(cluster=w1487, "Source Paths.CSS Files"=w1485, "Source Paths.JS Files"=w1484, "Source Paths.VI Template"=w1483, "Source Paths.Menu Template"=w1482, "Source Paths.PolyVI Template"=w1481) -> (w1479:T15)
            n739 = call "VIH Project - Container - Master Rule.vi"("cmd (get)"=enum16{"get", "set"}."set", "Rule in"=w1479) -> ()  [unwired: 9 in, 1 out]
          }
        }
        n740 = Concatenate Strings(w1472, w1476) -> (w1473:string)
      }
      frame "------------------------------- 4" {
      }
      frame "Tree: New" {
        (unwired) "Help Project\nProject Files\nBuild Help Rules"
        n741 = call "VIH UI - Get Icon 32x32 for Tree Item.vi"("cmd (get)"=enum16{"get", "reset"}."reset") -> ("error out"=w1492:errorcluster)  [unwired: 9 in, 1 out]
        n742 = invoke on="Tree" class="Tree (strict)" method="Edit Tree Items.Delete"(error in=w1492, "Delete Children"=TRUE) -> (error out=w1500:errorcluster)  [unwired: 3 in, 4 out]
        n743 = call "VIH Utility - STR - Constant String To Array.vi"("String in"="Help Project\nProject Files") -> ("Array out"=w1494:string[])  [unwired: 10 in]
        n744 = call "VIH Project Tree - Item Tag - Build.vi"("cmd (build)"=enum16{"build", "init"}."init", "Item Type"=VIH_Project_Tree_Typedef_-_Tree_Item_Type."<Invalid>") -> ("Tree Item Tag"=w1498:string)  [unwired: 8 in, 1 out]
        n745 = for {
          tunnel: w1494 -> [w1514] mode=indexing
          tunnel: w1498 -> [_]
          tunnel: w1500 -> [w1516]
          tunnel: [w1507] -> w1496
          i -> [w1513]
          n746 = case shown="0" w1513 {
            tunnel: [_ VIH_Project_Tree_Typedef_-_Tree_Item_Type."Project" ("Item Type") VIH_Project_Tree_Typedef_-_Tree_Item_Type."Proj Files" ("Item Type") VIH_Project_Tree_Typedef_-_Tree_Item_Type."Proj Rules" ("Item Type")] -> w1509
            tunnel: [_ _ VIH_Project_Tree_Typedef_-_Tree_Item_Type."Project" ("Item Type") VIH_Project_Tree_Typedef_-_Tree_Item_Type."Project" ("Item Type")] -> w1511
            frame Default {
            }
            frame 0 {
            }
            frame 1 {
            }
            frame 2 {
            }
          }
          n747 = call "VIH Project Tree - Item Tag - Build.vi"("Item Type"=w1511) -> ("Tree Item Tag"=w1510:string)  [unwired: 9 in, 1 out]
          n748 = call "VIH Project Tree - Item Tag - Build.vi"("Item Type"=w1509) -> ("Tree Item Symbol"=w1508:i32, "Tree Item Tag"=w1512:string)  [unwired: 9 in]
          n749 = call <vilib>:"Trim Whitespace.vi"("string"=w1514) -> ("trimmed string"=w1517:string)  [unwired: 1 in]
          n750 = invoke on="Tree" class="Tree (strict)" method="Edit Tree Items.Add Item"(error in=w1516, "Parent Tag"=w1510, "Child Position"=-1, "Left Cell"=w1517, "Child Tag"=w1512, "Child Only?"=FALSE) -> (error out=w1520:errorcluster, "Edit Tree Items:Add Item"=w1519:string)  [unwired: 3 in, 7 out]
          n751 = Empty String/Path?(string/path=w1510) -> (empty?=w1515:bool)
          n752 = property on="Tree" class="Tree (strict)"(error in=w1520, "Active Item Tag"=w1519, "Disabled?"=FALSE ("Active Item:Disabled?"), "Open?"=w1515, "Glyph"=w1508) -> (error out=w1507:errorcluster)  [unwired: 1 in, 1 out]
        }
        n753 = stacked-sequence {
          tunnel: w1496 -> [w1503]
          frame #0 {
            n754 = call "VIH Project Tree - Item Tag - Build.vi"("Item Type"=VIH_Project_Tree_Typedef_-_Tree_Item_Type."Project") -> ("Tree Item Tag"=w1505:string)  [unwired: 9 in, 1 out]
            n755 = Build Array(w1505) -> (w1504:string[])
            n756 = property on="Tree" class="Tree (strict)"(error in=w1503, "Value"=w1504) -> ()  [unwired: 1 in, 2 out]
          }
        }
      }
      frame "Tree: Build" {
        # "gather Icons (32x32) for project files"
        n757 = call "VIH UI - Get Icon 32x32 for Tree Item.vi"("cmd (get)"=enum16{"get", "reset"}."reset") -> ("error out"=w1533:errorcluster)  [unwired: 9 in, 1 out]
        n758 = control-ref of="Tree"() -> (w1535:refnum<vi>)
        n759 = call "VIH ProjFile - Core.vi"("error in"=w1533) -> ("error out"=w1550:errorcluster, "Project"=w1540:T36)  [unwired: 9 in]
        n760 = call "VIH Project - Container - Project File Path.vi"() -> ("Project File Path"=w1538:path)  [unwired: 9 in, 2 out]
        n761 = Strip Path(path=w1538) -> (stripped path=w1537:path)  [unwired: 1 out]
        n762 = Unbundle By Name(w1540) -> ("Files"=w1539:refnum<k20>)
        n763 = call "VIH Project Tree - Item Tag - Build.vi"("Item Type"=VIH_Project_Tree_Typedef_-_Tree_Item_Type."Project") -> ("Tree Item Tag"=w1546:string)  [unwired: 9 in, 1 out]
        n764 = call "VIH Project Tree - Item Tag - Build.vi"("Item Type"=VIH_Project_Tree_Typedef_-_Tree_Item_Type."Proj Files") -> ("Tree Item Tag"=w1545:string)  [unwired: 9 in, 1 out]
        n765 = call "VIH Project Tree - Item Tag - Build.vi"("Item Type"=VIH_Project_Tree_Typedef_-_Tree_Item_Type."Proj Rules") -> ("Tree Item Tag"=w1544:string)  [unwired: 9 in, 1 out]
        n766 = call "VIH ProjFile - File Tree - Read.vi"("Tree Parent Tag"=w1545, "Project Tree"=w1535, "error in"=w1550, "Project Folder"=w1537, "XML Parent Item"=w1539) -> ("error out"=w1536:errorcluster)  [unwired: 5 in, 1 out]
        n767 = call "VIH Project Tree - Sort Items.vi"("error in"=w1536, "Project Tree"=w1535) -> ("error out"=w1528:errorcluster)  [unwired: 7 in, 2 out]
        n768 = invoke on="Tree" class="Tree (strict)" method="Open/Close.Open/Close All"(error in=w1528, "Open"=FALSE) -> (error out=w1548:errorcluster)  [unwired: 2 in, 3 out]
        n769 = Build Array(w1546, w1545, w1544) -> (w1547:string[])
        n770 = for {
          tunnel: w1548 -> [w1558]
          tunnel: w1547 -> [w1556] mode=indexing
          tunnel: [w1555] -> w1531
          n771 = invoke on="Tree" class="Tree (strict)" method="Open/Close.Item"(error in=w1558, "tag"=w1556, "Open"=TRUE) -> (error out=w1555:errorcluster)  [unwired: 2 in, 4 out]
        }
        n772 = Bundle By Name(cluster=w1531, "status"=FALSE) -> (w1529:errorcluster)
        n773 = property on="Tree" class="Tree (strict)"(error in=w1529) -> ("All Tags"=w1532:string[])  [unwired: 1 in, 2 out]
        n774 = for {
          tunnel: w1532 -> [w1553] mode=indexing
          n775 = property on="Tree" class="Tree (strict)"("Active Item Tag"=w1553, "ActiveColNum"=0 ("Active Cell:Active Column Number")) -> ("Cell String"=w1552:string)  [unwired: 2 in, 2 out]
          n776 = call "VIH UI - Get Icon 32x32 for Tree Item.vi"("Item Name"=w1552, "Tree Item Tag"=w1553) -> ()  [unwired: 8 in, 2 out]
        }
      }
      frame "Tree: Sort" {
        n777 = Match Pattern(string=w1567, regular expression="\\s+?\\s+") -> (before substring=w1565:string, after substring=w1564:string)  [unwired: 1 in, 2 out]
        n778 = call <vilib>:"Trim Whitespace.vi"("string"=w1565) -> ("trimmed string"=w1563:string)  [unwired: 1 in]
        n779 = call <vilib>:"Trim Whitespace.vi"("string"=w1564) -> ("trimmed string"=w1560:string)  [unwired: 1 in]
        n780 = control-ref of="Tree"() -> (w1568:refnum<vi>)
        n781 = call "VIH Project Tree - Sort Items.vi"("Recursively (T)"=FALSE, "Parent Tag"=w1563, "Project Tree"=w1568) -> ("dup Project Tree"=w1562:T24)  [unwired: 6 in, 2 out]
        n782 = Empty String/Path?(string/path=w1560) -> (empty?=w1561:bool)
        n783 = call "VIH Project - Change Flag.vi"("cmd (get)"=enum16{"get", "set", "reset"}."set") -> ()  [unwired: 9 in, 2 out]
        n784 = case shown="False" w1561 {
          tunnel: w1562 -> [w1572 _]
          tunnel: w1560 -> [w1571 _]
          frame False {
            n785 = invoke class="Tree (strict)" method="Open/Close.Ensure Visible"(reference=w1572, "tag"=w1571) -> ()  [unwired: 2 in, 4 out]
          }
          frame True {
          }
        }
      }
      frame "Tree: Check" {
        n786 = control-ref of="Tree"() -> (w1574:refnum<vi>)
        n787 = call "VIH Project Tree - Create Unique Output Names for Added Files.vi"("Check All (F)"=TRUE, "Added Item Tags"=string[] [], "Project Tree"=w1574) -> ("dup Project Tree"=w1573:T24)  [unwired: 7 in, 1 out]
        n788 = call "VIH Project Tree - Find Invalid Files in Project Tree.vi"("Project Tree"=w1573) -> ("Tree Item Tags"=w1577:string[])  [unwired: 7 in, 3 out]
        n789 = Empty Array?(array=w1577) -> (empty?=w1581:bool)
        n790 = case shown="False" w1581 {
          tunnel: w1577 -> [w1590 _]
          tunnel: ["Defer FP Update = ON;\nUpdate Controls;\nDefer FP Update = OFF;\n\nKey Focus = Tree;" _] -> w1579
          tunnel: [w1585 _] -> w1578
          frame False {
            n791 = for {
              tunnel: w1590 -> [w1594] mode=indexing
              tunnel: [w1593] -> w1583
              n792 = invoke on="Tree" class="Tree (strict)" method="Open/Close.Ensure Visible"("tag"=w1594) -> (error out=w1593:errorcluster)  [unwired: 3 in, 3 out]
            }
            n793 = stacked-sequence {
              tunnel: "WARNING:\nSome project files could not be found!\n\nWould you like to review missed files?" ("format string") -> [w1592]
              tunnel: [w1591] -> w1587
              tunnel: w1583 -> [_]
              frame #0 {
                n794 = Two Button Dialog(message=w1592) -> (T button?=w1591:bool)  [unwired: 2 in]
              }
            }
            n795 = Select(t="Menu = File List ? Invalid;", s=w1587, f="") -> (s? t:f=w1585:string)
          }
          frame True {
          }
        }
        n796 = Concatenate Strings(w1579, w1578, w1582) -> (w1580:string)
      }
      frame "------------------------------- 5" {
      }
      frame "Update Window Title" {
        n797 = call "VIH Project - Container - Project File Path.vi"() -> ("Project File Path"=w1602:path)  [unwired: 9 in, 2 out]
        n798 = Empty String/Path?(string/path=w1602) -> (empty?=w1604:bool)
        n799 = call "VIH Project - Change Flag.vi"() -> ("Flag"=w1600:bool)  [unwired: 10 in, 1 out]
        n800 = case shown="False" w1604 {
          tunnel: w1602 -> [w1610 _]
          tunnel: w1601 -> [w1609 w1611]
          tunnel: [w1607 w1611] -> w1603
          frame False {
            n801 = Strip Path(path=w1610) -> (name=w1608:string)  [unwired: 1 out]
            n802 = Format Into String(format string=" - %s", initial string=w1609, w1608) -> (resulting string=w1607:string)  [unwired: 1 in, 1 out]
          }
          frame True {
          }
        }
        n803 = Select(t=" *", s=w1600, f="") -> (s? t:f=w1596:string)
        n804 = Concatenate Strings(w1603, w1596) -> (w1597:string)
        n805 = property class="VI"("Front Panel.Title"=w1597) -> ()  [unwired: 2 in, 2 out]
      }
      frame "Update Controls" {
        n806 = control-ref of="Sub Panel"() -> (w1620:refnum<vi>)
        n807 = control-ref of="Tree"() -> (w1618:refnum<vi>)
        n808 = call "VIH UI - Tree Value Changed.vi"("SubPanel"=w1620, "Project Tree"=w1618) -> ("Item Title"=→"Item Title":string, "Item Icon"=→"Item Icon":picture, "dup Tree Refnum"=w1617:T24)  [unwired: 6 in, 1 out]
        n809 = case shown="\"INIT\"" w1616 {
          tunnel: w1617 -> [_ w1626]
          tunnel: [_ w1622] -> _
          frame Default {
          }
          frame "INIT" {
            n810 = Build Array("General") -> (w1623:string[])
            n811 = call "VIH UI - Controller for Property Pages.vi"("cmd (update)"=T5."Set Category", "Params"=w1623, "Project Tree"=w1626) -> ("error out"=w1622:errorcluster)  [unwired: 7 in, 1 out]
          }
        }
        n812 = Concatenate Strings("Update Toolbar;", w1621) -> (w1615:string)
        "Item Icon BG" <- ""
      }
      frame "Update Toolbar" {
        n813 = Index Array(array=w1655) -> (element=w1659:string)  [unwired: 1 in]
        n814 = control-ref of="Tree"() -> (w1664:refnum<vi>)
        n815 = Array Size(array=w1655) -> (size(s)=w1654:i32)
        n816 = call "VIH Project Tree - Item Tag - Parse.vi"("Tree Item Tag"=w1659) -> ("Item File Path"=w1650:path, "Item Type"=w1651:T2)  [unwired: 8 in, 1 out]
        n817 = Equal?(x=w1654, y=1) -> (x = y?=w1652:bool)
        n818 = In Range and Coerce(upper limit=VIH_Project_Tree_Typedef_-_Tree_Item_Type."Proj Rules" ("Item Type"), x=w1651, lower limit=VIH_Project_Tree_Typedef_-_Tree_Item_Type."Project" ("Item Type")) -> (In Range?=w1656:bool)  [unwired: 1 out]
        n819 = case shown="False" w1656 {
          tunnel: w1664 -> [w1681 w1714]
          tunnel: [w1685 _] -> w1663
          tunnel: [w1684 w1714] -> w1662
          tunnel: w1655 -> [w1672 _]
          tunnel: w1652 -> [w1675 _]
          tunnel: w1651 -> [w1668 _]
          tunnel: w1650 -> [w1683 _]
          tunnel: [w1680 _] -> w1649
          tunnel: [w1677 _] -> w1644
          tunnel: [w1674 _] -> w1635
          tunnel: [w1671 _] -> w1640
          tunnel: [w1669 _] -> w1639
          tunnel: [w1667 _] -> w1629
          frame False {
            n820 = call "VIH Project Tree - Item Type to Boolean Flags (extra #1).vi"("Item Type"=w1668) -> ("Can be documented"=w1667:bool)  [unwired: 9 in, 1 out]
            n821 = call "VIH Project Tree - Item Type to Boolean Flags.vi"("Item Type"=w1668) -> ("VI with Conpane"=w1678:bool, "Can be built"=w1679:bool, "Can be opened"=w1676:bool)  [unwired: 4 in, 4 out]
            n822 = for {
              tunnel: [w1690] -> w1673 mode=indexing
              tunnel: w1672 -> [w1689] mode=indexing
              tunnel: [w1686] -> w1670 mode=indexing
              n823 = call "VIH Project Tree - Item Tag - Parse.vi"("Tree Item Tag"=w1689) -> ("Item File Path"=w1688:path, "Item Type"=w1691:T2)  [unwired: 8 in, 1 out]
              n824 = Empty String/Path?(string/path=w1688) -> (empty?=w1687:bool)
              n825 = call "VIH Project Tree - Item Type to Boolean Flags.vi"("Item Type"=w1691) -> ("Can be Removed"=w1690:bool)  [unwired: 4 in, 6 out]
              n826 = Not(x=w1687) -> (.not. x?=w1686:bool)
            }
            n827 = And(x=w1675, y=w1678) -> (x .and. y?=w1677:bool)
            n828 = And(x=w1679, y=w1675) -> (x .and. y?=w1682:bool)
            n829 = And(x=w1676, y=w1675) -> (x .and. y?=w1674:bool)
            n830 = case shown="True" w1682 {
              tunnel: [_ w1704] -> w1680
              tunnel: w1681 -> [_ w1707]
              tunnel: w1668 -> [_ w1706]
              tunnel: w1683 -> [_ w1705]
              frame False {
              }
              frame True {
                n831 = call "VIH Project - Get Effective File Rule.vi"("Ignore Control Rules (F)"=TRUE, "File Path"=w1705, "Project Tree"=w1707) -> ("Effective File Rule"=w1708:T30)  [unwired: 5 in, 3 out]
                n832 = Unbundle By Name(w1708) -> ("Target Paths.HTML Dir"=w1711:path, "OutName"=w1710:string)
                n833 = call "VIH Project Tree - Item Type to Palette Item Type.vi"("Tree Item Type"=w1706) -> ("Item/File Type"=w1713:T33)  [unwired: 9 in, 1 out]
                n834 = call "VIH HelpGen - Get Target HTML Filename.vi"("Item File Path"=w1705, "Item Type"=w1713, "HTML Filename in"=w1710) -> ("HTML Fileame out"=w1712:string)  [unwired: 7 in, 1 out]
                n835 = Build Path(base path=w1711, name or relative path=w1712) -> (appended path=w1703:path)
                n836 = call "VIH HelpGen - FILE - Check File Path (Buffered).vi"("Force Update (T)"=FALSE, "File Path"=w1703) -> ("Good path"=w1704:bool)  [unwired: 8 in, 1 out]
              }
            }
            n837 = case shown="False" w1679 {
              selector: w1679 -> [_ w1700]
              tunnel: [w1695 w1700] -> w1685
              tunnel: [w1694 w1701] -> w1684
              tunnel: w1672 -> [w1693 _]
              tunnel: w1681 -> [w1692 w1701]
              frame False {
                n838 = for {
                  tunnel: w1693 -> [w1698] mode=indexing
                  tunnel: [w1697] -> w1695
                  shift-right: [w1696] -> w1694
                  shift-left: w1692 -> [w1699]
                  stop <- w1697 stop-if-true
                  n839 = call "VIH Project Tree - Can Items Be Built.vi"("Parent Item Tag (Root)"=w1698, "Project Tree"=w1699) -> ("Can be built"=w1697:bool, "dup Project Tree"=w1696:T24)  [unwired: 6 in, 2 out]
                }
              }
              frame True {
              }
            }
            n840 = And Array Elements(Boolean array=w1673) -> (logical AND=w1671:bool)
            n841 = And Array Elements(Boolean array=w1670) -> (logical AND=w1669:bool)
          }
          frame True {
          }
        }
        n842 = call "VIH Project - Container - HHP Generation.vi"() -> ("HHP_Generation out"=w1634:T34)  [unwired: 11 in]
        n843 = call "VIH - CHM Project - Get Actual HHP_Generation Params.vi"("HHP_Generation"=w1634) -> ("CHM File Absolute Path"=w1632:path)  [unwired: 8 in, 2 out]
        n844 = call "VIH HelpGen - FILE - Check File Path (Buffered).vi"("Force Update (T)"=FALSE, "File Path"=w1632) -> ("Good path"=w1631:bool)  [unwired: 8 in, 1 out]
        n845 = call "VIH Utility - UI - Boolean to Control Disable Status.vi"("Status in"=w1631) -> ("Control Disable if False"=w1630:u8)  [unwired: 3 in, 1 out]
        n846 = property on="%Toolbar_BuildCHMOpen" class="Bool"("DisabledEnum"=w1630) -> ()  [unwired: 2 in, 2 out]
        n847 = call "VIH Project - Container - Project File Path.vi"() -> ("Project Build Log File"=w1647:path)  [unwired: 9 in, 2 out]
        n848 = case shown="False" w1663 {
          selector: w1663 -> [_ w1717]
          tunnel: w1662 -> [w1716 _]
          tunnel: [w1715 w1717] -> w1661
          frame False {
            n849 = call "VIH Project Tree - Can Items Be Built.vi"("Project Tree"=w1716) -> ("Can be built"=w1715:bool)  [unwired: 7 in, 3 out]
          }
          frame True {
          }
        }
        n850 = call "VIH Utility - UI - Boolean to Control Disable Status.vi"("Status in"=w1640) -> ("Control Disable if False"=w1641:u8)  [unwired: 3 in, 1 out]
        n851 = call "VIH Utility - UI - Boolean to Control Disable Status.vi"("Status in"=w1639) -> ("Control Disable if False"=w1638:u8)  [unwired: 3 in, 1 out]
        n852 = call "VIH Utility - UI - Boolean to Control Disable Status.vi"("Status in"=w1635) -> ("Control Disable if False"=w1642:u8)  [unwired: 3 in, 1 out]
        n853 = call "VIH Utility - UI - Boolean to Control Disable Status.vi"("Status in"=w1635) -> ("Control Disable if False"=w1636:u8)  [unwired: 3 in, 1 out]
        n854 = call "VIH Utility - UI - Boolean to Control Disable Status.vi"("Status in"=w1649) -> ("Control Disable if False"=w1648:u8)  [unwired: 3 in, 1 out]
        n855 = call "VIH Utility - UI - Boolean to Control Disable Status.vi"("Status in"=w1644) -> ("Control Disable if False"=w1643:u8)  [unwired: 3 in, 1 out]
        n856 = call "VIH Utility - UI - Boolean to Control Disable Status.vi"("Status in"=w1629) -> ("Control Disable if False"=w1628:u8)  [unwired: 3 in, 1 out]
        n857 = call "VIH HelpGen - FILE - Check File Path (Buffered).vi"("Force Update (T)"=FALSE, "File Path"=w1647) -> ("Good path"=w1646:bool)  [unwired: 8 in, 1 out]
        n858 = property on="%Toolbar_Delete" class="Bool"("DisabledEnum"=w1641) -> ()  [unwired: 2 in, 2 out]
        n859 = property on="%Toolbar_Copy" class="Bool"("DisabledEnum"=w1638) -> ()  [unwired: 2 in, 2 out]
        n860 = property on="%Toolbar_VI_Open" class="Bool"("DisabledEnum"=w1642) -> ()  [unwired: 2 in, 2 out]
        n861 = property on="%Toolbar_VI_Edit" class="Bool"("DisabledEnum"=w1636) -> ()  [unwired: 2 in, 2 out]
        n862 = property on="%Toolbar_BuildOpen" class="Bool"("DisabledEnum"=w1648) -> ()  [unwired: 2 in, 2 out]
        n863 = property on="%Toolbar_VI_Term" class="Bool"("DisabledEnum"=w1643) -> ()  [unwired: 2 in, 2 out]
        n864 = property on="%Toolbar_VI_Doc" class="Bool"("DisabledEnum"=w1628) -> ()  [unwired: 2 in, 2 out]
        n865 = call "VIH Utility - UI - Boolean to Control Disable Status.vi"("Status in"=w1646) -> ("Control Disable if False"=w1637:u8)  [unwired: 3 in, 1 out]
        n866 = call "VIH Utility - UI - Boolean to Control Disable Status.vi"("Status in"=w1661) -> ("Control Disable if False"=w1660:u8)  [unwired: 3 in, 1 out]
        n867 = call "VIH Utility - UI - Boolean to Control Disable Status.vi"("Status in"=w1663) -> ("Control Disable if False"=w1665:u8)  [unwired: 3 in, 1 out]
        n868 = property on="%Toolbar_BuildLog" class="Bool"("DisabledEnum"=w1637) -> ()  [unwired: 2 in, 2 out]
        n869 = property on="%Toolbar_BuildCHM" class="Bool"("DisabledEnum"=T12."Enabled" ("Disabled")) -> ()  [unwired: 2 in, 2 out]
        n870 = property on="%Toolbar_BuildAll" class="Bool"("DisabledEnum"=w1660) -> ()  [unwired: 2 in, 2 out]
        n871 = property on="%Toolbar_BuildSel" class="Bool"("DisabledEnum"=w1665) -> ()  [unwired: 2 in, 2 out]
      }
      frame "Update Toolbar: Warning" {
        n872 = control-ref of="Tree"() -> (w1736:refnum<vi>)
        n873 = To Lower Case(string=w1725) -> (all lower case string=w1723:string)
        n874 = call "VIH Project Tree - Find Invalid Files in Project Tree.vi"("Project Tree"=w1736) -> ("Item Paths"=w1734:path[], "dup Project Tree"=w1735:T24)  [unwired: 7 in, 2 out]
        n875 = Equal?(x=w1723, y="dialog") -> (x = y?=w1722:bool)
        n876 = Empty Array?(array=w1734) -> (empty?=w1733:bool)
        n877 = case shown="True" w1733 {
          selector: w1733 -> [w1742 _]
          tunnel: w1735 -> [_ w1745]
          tunnel: [w1742 w1743] -> w1731
          frame False {
          }
          frame True {
            n878 = call "VIH Project Tree - Find Lost Item Rules.vi"("Project Tree"=w1745) -> ("Lost Rules (Owner Paths)"=w1744:path[])  [unwired: 8 in, 2 out]
            n879 = Empty Array?(array=w1744) -> (empty?=w1743:bool)
          }
        }
        n880 = call "VIH Project - Verify CSS,JS,Template Files.vi"() -> ("error"=w1730:bool)  [unwired: 9 in, 2 out]
        n881 = call "VIH Utility - UI - Boolean to Control Disable Status.vi"("Status in"=w1730) -> ("Control Disable if False"=w1728:u8)  [unwired: 3 in, 1 out]
        n882 = call "VIH Utility - UI - Boolean to Control Disable Status.vi"("Status in"=w1731) -> ("Control Disable if True"=w1729:u8)  [unwired: 3 in, 1 out]
        n883 = Max & Min(x=w1729, y=w1728) -> (min(x,y)=w1727:u8)  [unwired: 1 out]
        n884 = Equal To 0?(x=w1727) -> (x = 0?=w1726:bool)
        n885 = property on="%Toolbar_Warning" class="Bool"("DisabledEnum"=w1727) -> ()  [unwired: 2 in, 2 out]
        n886 = And(x=w1722, y=w1726) -> (x .and. y?=w1721:bool)
        n887 = case shown="True" w1721 {
          tunnel: "WARNING!!!\nThis project refers to some source files that could not be found (they may have been removed or renamed).\n\nClick OK to start review of missed files." -> [_ w1741]
          tunnel: [_ w1737] -> w1718
          frame False {
          }
          frame True {
            n888 = Two Button Dialog(message=w1741) -> (T button?=w1740:bool)  [unwired: 2 in]
            n889 = Select(t="Menu = WARNING;", s=w1740, f="") -> (s? t:f=w1737:string)
          }
        }
        n890 = Concatenate Strings(w1732, w1718) -> (w1719:string)
      }
    }
  }
